vi "ReversedEngineering GetClassDependencyInfo.vi"(1 "Class/Create Path":path=path "C:/classes/P1S/EG1_class/EG1.lvclass", 5 "error in (no error)":errorcluster, 6 "AttributeSerachP{atternNamesToIgnore":string[](array[string]), 7 "Only analyse this class methods and attributes(False)":bool) -> (15 "classInfo":T5, 16 "TypeDefs":T1[](array[typedef]), 19 "error out":errorcluster)   [LabVIEW 2020]
doc: "Gets current diagram values"
uses:
  <resource>/Framework/Providers/Open_GDS/UML/ReversedEngineering/ReversedEngineering ClassInfoType.ctl
  <resource>/Framework/Providers/Open_GDS/ClassProviders/Common/CommonVIs/CommonVIs_VisibilityType.ctl
  <resource>/Framework/Providers/Open_GDS/ClassProviders/Common/CommonVIs/CommonVIs_AttributeInfoType.ctl
  <resource>/Framework/Providers/Open_GDS/ClassProviders/Common/CommonVIs/CommonVIs_AttributeDataType.ctl
  <resource>/Framework/Providers/Open_GDS/UML/ReversedEngineering/ReversedEngineering_ClassDependencyDetailsType.ctl
  <resource>/Framework/Providers/Open_GDS/ClassProviders/Common/ScriptingFunctions/SubVIs/Scripting_ViDependencyType.ctl
  <resource>/Framework/Providers/Open_GDS/ClassProviders/Common/CommonVIs/CommonVIs_TypeDefType.ctl
  <resource>/Framework/Providers/Open_GDS/ClassProviders/Provider_BaseClassInterface/ClassReader_class/MethodDependencyType.ctl
  <resource>/Framework/Providers/Open_GDS/UML/UMLEditor/UMLEditor BusyDialogAction.ctl
  <resource>/Framework/Providers/Open_GDS/ClassProviders/Provider_BaseClassInterface/ClassReader_class/ClassReader.lvclass
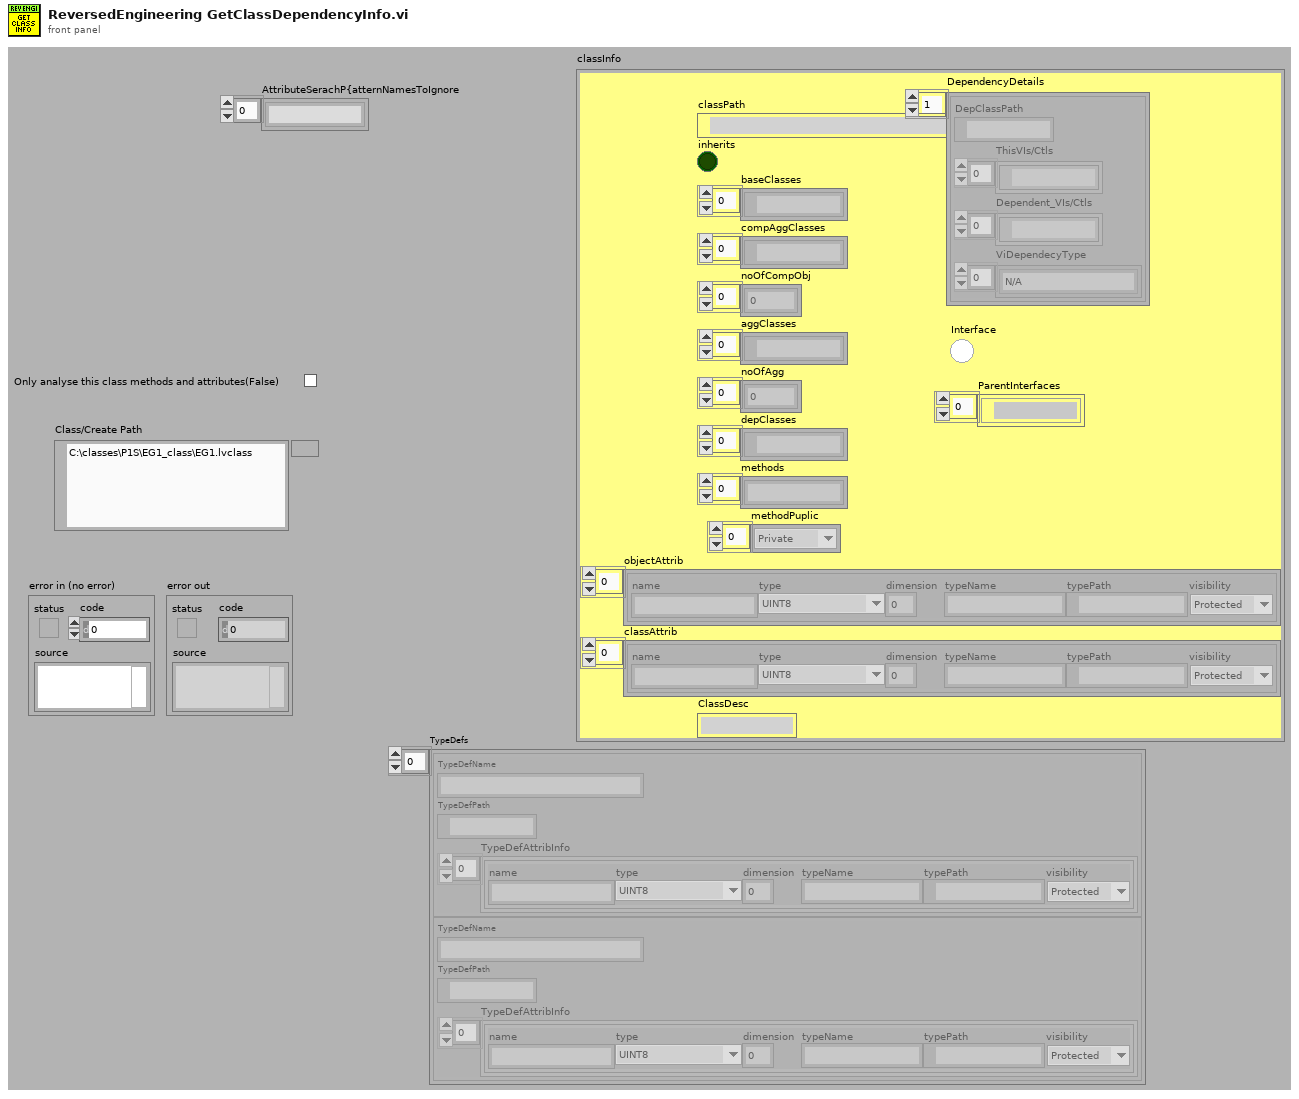
[diagram p1: front panel]
types:
  T1 = typedef "CommonVIs_TypeDefType.ctl" = cluster{"TypeDefName":string, "TypeDefPath":path, "TypeDefAttribInfo":T2[]}
  T2 = typedef "CommonVIs_AttributeInfoType.ctl" = cluster{"name":string, "type":T3, "dimension":i32, "typeName":string, "typePath":path, "visibility":T4}
  T3 = typedef "CommonVIs_AttributeDataType.ctl" = enum16{"UINT8", "INT8", "UINT16", "INT16", "UINT32", "INT32", "UINT64", "INT64", "SGL", "DBL", "EXT", "CSG", "CDB", "CXT", "TimeStamp", "STRING", "PATH", "BOOL", "ENUM", "RefNum", "VIRefNum", "LabVIEW Class", "Cluster", "Variant", "TypeDef", "Waveform", "LabVIEW Object", "Other", "void", "Set", "Map"}
  T4 = typedef "CommonVIs_VisibilityType.ctl" = enum16{"Public", "Private", "Protected"}
  T5 = typedef "ReversedEngineering ClassInfoType.ctl" = cluster{"classPath":path, "inherits":bool, "baseClasses":path[], "compAggClasses":path[], "noOfCompObj":i32[], "aggClasses":path[], "noOfAgg":i32[], "depClasses":path[], "methods":string[], "methodPuplic":T4[], "objectAttrib":T2[], "classAttrib":T2[], "ClassDesc":string, "DependencyDetails":T6[], "Interface":bool, "ParentInterfaces":path[]}
  T6 = typedef "ReversedEngineering_ClassDependencyDetailsType.ctl" = cluster{"DepClassPath":path, "ThisVIs/Ctls":path[], "Dependent_VIs/Ctls":path[], "ViDependecyType":T7[]}
  T7 = typedef "Scripting_ViDependencyType.ctl" = enum16{"N/A", "Launches"}
  T8 = typedef "ClassReader.lvclass/MethodDependencyType.ctl" = cluster{"Method/VI":path, "SubVIs/Ctls":path[], "SubVIClassOwner":string[], "ClassMethodName":string[], "SubVIClassOwnerPath":path[], "DepType":T7[]}
  T9 = cluster{"inherits":bool, "baseClasses":path[], "compositeAggregationClassPath":path[], "noOfCompositeObjects":i32[], "aggregationClassPath":path[], "noOfAggObjects":i32[], "dependencyClassPath":path[], "className":string, "classPath":path, "createRef":refnum<vi>, "depClassDescRefs":refnum<vi>[], "createPath":path, "depClassNames":string[], "depClassPaths":path[], "noOfObjects1":i32[], "refData":string, "refType":i16[], "noOfObjects2":i32[], "depTypeDefsVIs":path[], "depTypeDefsClassPath":path[], "depCreateClassPaths":path[], "objectRefsInAttrib":path[], "objectRefClassesInAttrib":path[], "objectRefInAttribIsAnArray":bool[], "methodNames":string[], "objectAttribInfo":T2[], "classAttribInfo":T2[], "errMsg":string, "dirClass":bool, "CreateClassVIsCalled":path[], "TypeDefs":T1[], "ClassDesc":string, "DependencyDetails":T6[], "methodPuplic":T4[], "depMethodVIs":T8[], "DataFlowClass":bool, "IsDependencyClassPathsAByValueClass":bool[], "Interface":bool, "ParentInterfaces":path[]}
  T10 = typedef "UMLEditor BusyDialogAction.ctl" = enum16{"Initialize", "Open(VIs)", "Open(i)", "Send_I-Value", "SendStatusMessage", "GetBusyDialogStatus", "Close", "Quit"}
  T11 = enum16{"NormalSubVis", "LV-Internal VIs", "All VIs", "All Functions"}
  T12 = enum32{"invalid VI type", "Standard VI", "Control VI", "Global VI", "Polymorphic VI", "Configuration VI", "SubSystem", "Facade VI", "Method VI", "Statechart Diagram VI"}
  T13 = enum32{"invalid scope", "public", "private", "protected", "community"}
  T14 = typedef "ClassTypes_MethodType.ctl" = cluster{"MethodName":string, "Visibility":enum16{"Public", "Private", "Protected"}, "StereoType":string, "Path":path}
  T15 = typedef "Librarian File Info Out.ctl" = cluster{"creation date":u32, "last mod date":u32, "type":string, "creator":string, "LV version":i32, "size":i32, "top level":bool}
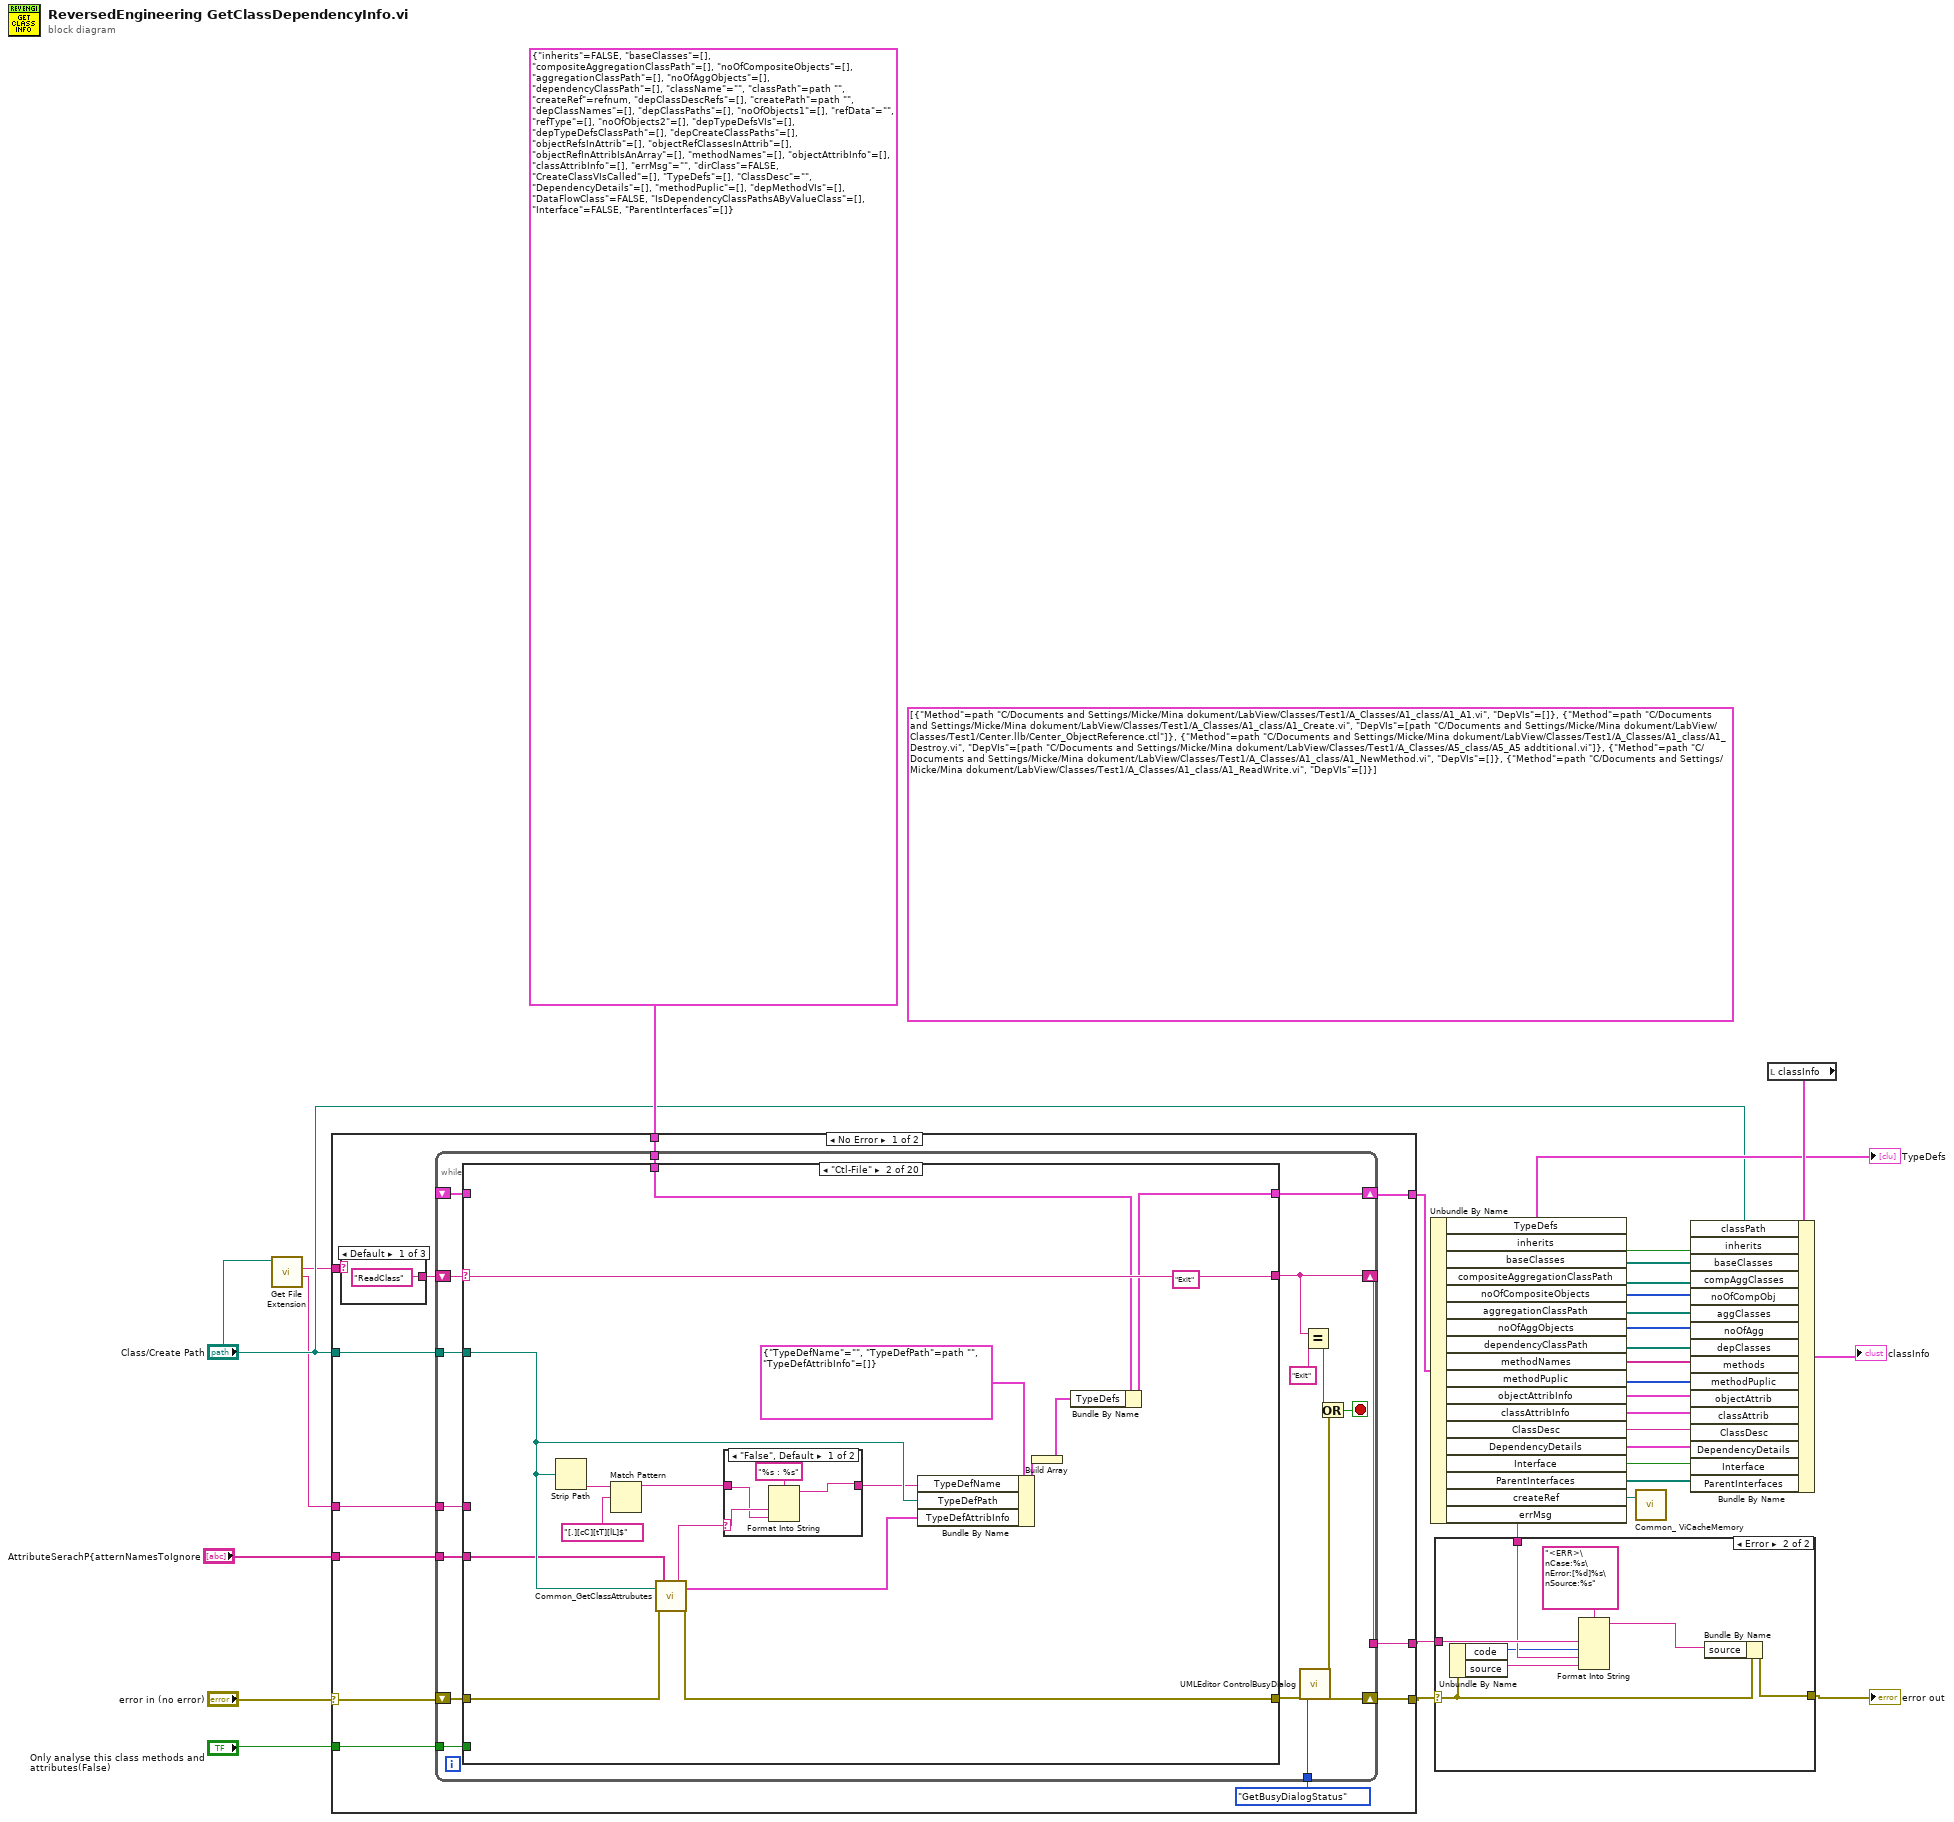
[diagram p0: block diagram]
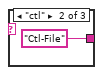
[diagram p3: hidden frame]
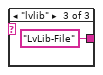
[diagram p4: hidden frame]
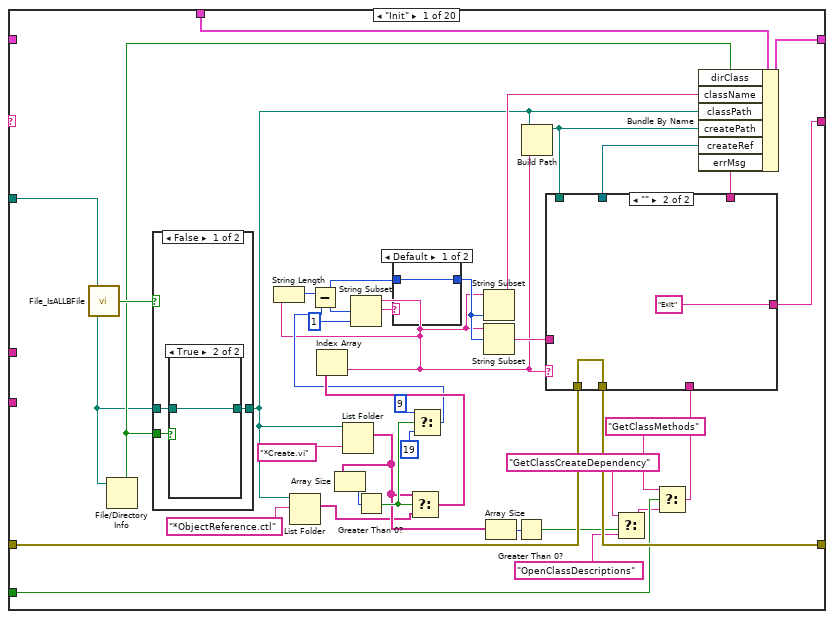
[diagram p5: hidden frame]
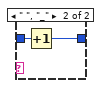
[diagram p6: hidden frame]
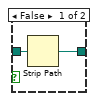
[diagram p7: hidden frame]
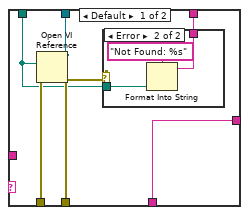
[diagram p9: hidden frame]
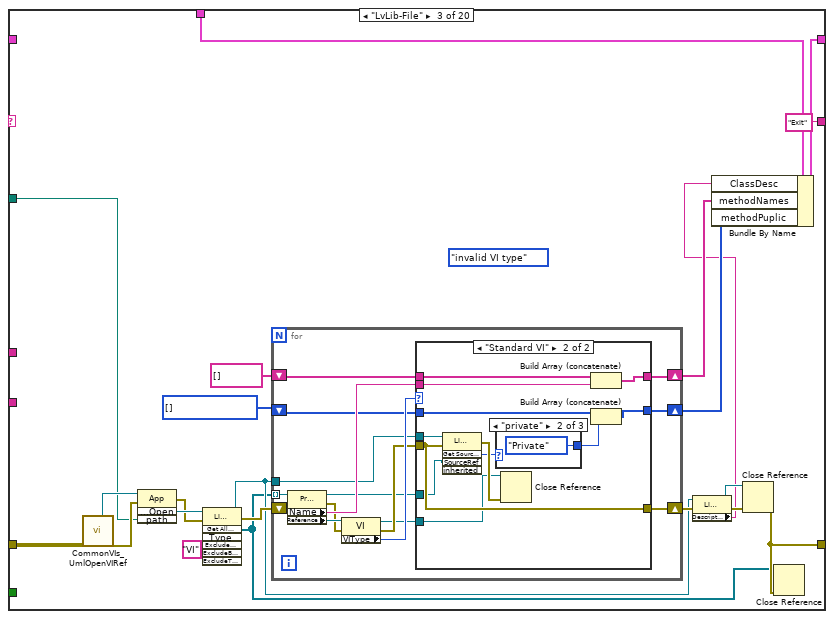
[diagram p12: hidden frame]
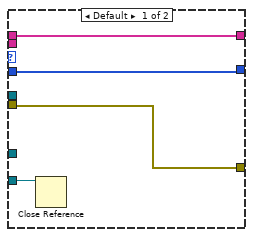
[diagram p13: hidden frame]
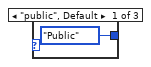
[diagram p14: hidden frame]
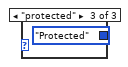
[diagram p15: hidden frame]
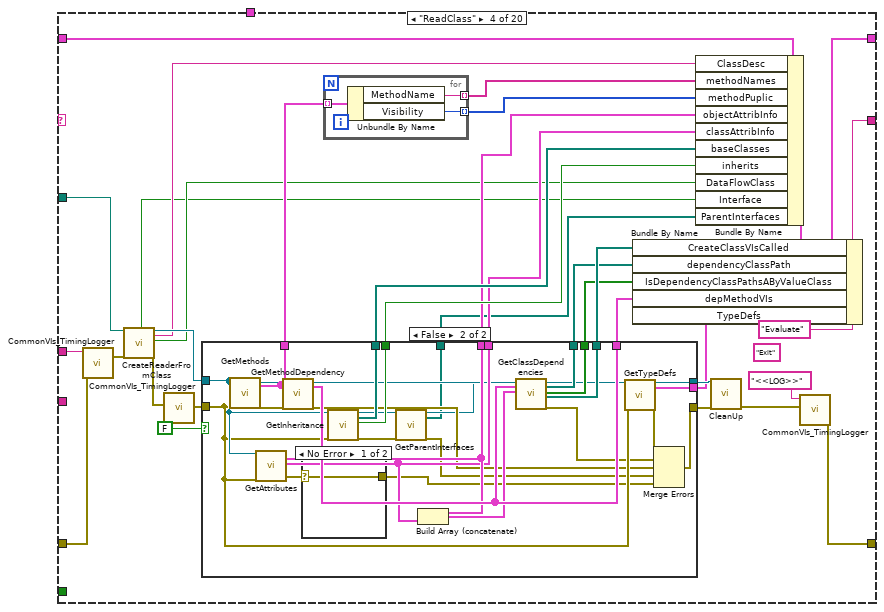
[diagram p16: hidden frame]
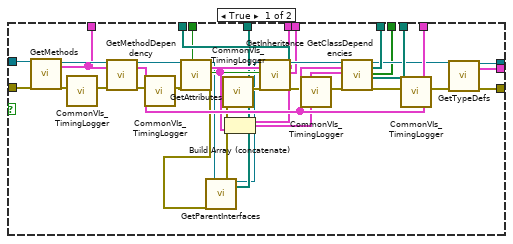
[diagram p17: hidden frame]
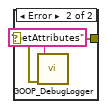
[diagram p18: hidden frame]
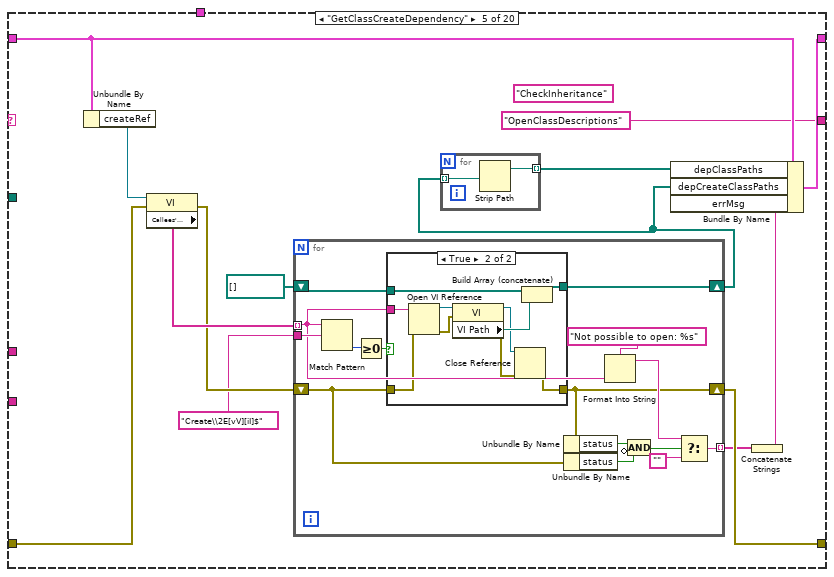
[diagram p19: hidden frame]
diagram:
  (unwired) cluster{"Method":path, "DepVIs":path[]}[] [{"Method"=path "C:/Documents and Settings/Micke/Mina dokument/LabView/Classes/Test1/A_Classes/A1_class/A1_A1.vi", "DepVIs"=[]}, {"Method"=path "C:/Documents and Settings/Micke/Mina dokument/LabView/Classes/Test1/A_Classes/A1_class/A1_Create.vi", "DepVIs"=[path "C:/Documents and Settings/Micke/Mina dokument/LabView/Classes/Test1/Center.llb/Center_ObjectReference.ctl"]}, {"Method"=path "C:/Documents and Settings/Micke/Mina dokument/LabView/Classes/Test1/A_Classes/A1_class/A1_Destroy.vi", "DepVIs"=[path "C:/Documents and Settings/Micke/Mina dokument/LabView/Classes/Test1/A_Classes/A5_class/A5_A5 addtitional.vi"]}, {"Method"=path "C:/Documents and Settings/Micke/Mina dokument/LabView/Classes/Test1/A_Classes/A1_class/A1_NewMethod.vi", "DepVIs"=[]}, {"Method"=path "C:/Documents and Settings/Micke/Mina dokument/LabView/Classes/Test1/A_Classes/A1_class/A1_ReadWrite.vi", "DepVIs"=[]}] ("depMethodVIs")
  n1 = call <vilib>:"Get File Extension.vi"("file"="Class/Create Path") -> ("filename without extension"=w4:string, "lowercase file extension"=w5:string)  [unwired: 1 in, 8 out]
  n2 = case shown="No Error" "error in (no error)" {
    selector: "error in (no error)" -> [w43 w1104]
    tunnel: [w42 w1104] -> w16
    tunnel: "Class/Create Path" -> [w41 _]
    tunnel: [w40 _] -> w30
    tunnel: [w39 _] -> w14
    tunnel: "Only analyse this class methods and attributes(False)" -> [w38 _]
    tunnel: T9 {"inherits"=FALSE, "baseClasses"=[], "compositeAggregationClassPath"=[], "noOfCompositeObjects"=[], "aggregationClassPath"=[], "noOfAggObjects"=[], "dependencyClassPath"=[], "className"="", "classPath"=path "", "createRef"=refnum, "depClassDescRefs"=[], "createPath"=path "", "depClassNames"=[], "depClassPaths"=[], "noOfObjects1"=[], "refData"="", "refType"=[], "noOfObjects2"=[], "depTypeDefsVIs"=[], "depTypeDefsClassPath"=[], "depCreateClassPaths"=[], "objectRefsInAttrib"=[], "objectRefClassesInAttrib"=[], "objectRefInAttribIsAnArray"=[], "methodNames"=[], "objectAttribInfo"=[], "classAttribInfo"=[], "errMsg"="", "dirClass"=FALSE, "CreateClassVIsCalled"=[], "TypeDefs"=[], "ClassDesc"="", "DependencyDetails"=[], "methodPuplic"=[], "depMethodVIs"=[], "DataFlowClass"=FALSE, "IsDependencyClassPathsAByValueClass"=[], "Interface"=FALSE, "ParentInterfaces"=[]} ("Cluster") -> [w36 _]
    tunnel: w5 -> [w35 _]
    tunnel: w4 -> [w33 _]
    tunnel: "AttributeSerachP{atternNamesToIgnore" -> [w32 _]
    frame No Error {
      n3 = case shown="Default" w35 {
        tunnel: ["ReadClass" ("y") "Ctl-File" "LvLib-File"] -> w34
        frame Default {
        }
        frame "ctl" {
        }
        frame "lvlib" {
        }
      }
      n4 = while {
        shift-right: [w61] -> _
        shift-left: w34 -> [w54]
        shift-right: [w48] -> w42
        shift-left: w43 -> [w62]
        shift-right: [w56] -> w40
        shift-left: _ -> [w57]
        tunnel: w41 -> [w55]
        tunnel: [w54] -> w39
        tunnel: w38 -> [w53]
        tunnel: UMLEditor_BusyDialogAction."GetBusyDialogStatus" ("Action(SendStatusMessage)") -> [w51]
        tunnel: w36 -> [w50]
        tunnel: w33 -> [w49]
        tunnel: w32 -> [w47]
        stop <- w58 stop-if-true
        n5 = case shown="\"Ctl-File\"" w54 {
          tunnel: w62 -> [w90 w137 w160 w206 w310 w344 w372 w437 w483 w579 w665 w685 w707 w730 w795 w817 w883 w958 w1022 w1101]
          tunnel: [w89 w135 w144 w200 w306 w340 w373 w437 w464 w579 w670 w698 w705 w730 w795 w817 w883 w958 w1022 w1101] -> w52
          tunnel: [w99 "Exit" ("y") "Exit" ("y") "Evaluate" ("y") "OpenClassDescriptions" ("y") "CheckInheritance" ("y") "GetMultiplicity" ("y") "GetClassMethods" ("y") "GetClassMethodDepenencies" ("y") "GetObjectAttributsDepenencies" ("y") "GetClassAttributsDepenencies" ("y") "CloseRefs" ("y") "Evaluate" ("y") "RemoveInheritDependency" ("y") "CreateTypeDefs?" ("y") "AddReferencedTypeDefs" ("y") "UpdateTypeDefsAttribName?" ("y") "SortMethodToClassDependencies" ("y") "Exit" ("y") "Exit" ("y")] -> w61
          tunnel: w57 -> [_ _ _ w229 w305 w362 w369 w440 w478 w575 w672 w693 w706 w714 w793 w812 w885 w965 w1021 w1103]
          tunnel: [w98 w134 w162 w220 w304 w363 w377 w442 w479 w580 w673 w694 w706 w729 w794 w819 w884 w964 w1023 w1103] -> w56
          tunnel: w55 -> [w71 w130 w159 w230 _ _ _ _ _ _ _ _ _ _ _ _ _ _ _ _]
          tunnel: w53 -> [w74 _ _ _ _ _ _ _ _ _ _ _ _ _ _ _ _ _ _ _]
          tunnel: w50 -> [w63 w126 w145 _ _ _ _ _ _ _ _ _ _ _ _ _ _ _ _ _]
          tunnel: w49 -> [_ _ _ w205 _ _ _ _ _ _ _ _ _ _ _ _ _ _ _ _]
          tunnel: w47 -> [_ w122 _ _ _ _ _ _ _ _ _ _ _ _ _ _ _ _ _ _]
          frame "Init" {
            n6 = call <resource>:"File_IsALLBFile.vi"("path"=w71) -> ("path to VI library?"=w100:bool)
            n7 = File/Directory Info(path=w71) -> (directory=w87:bool)  [unwired: 1 in, 6 out]
            n8 = case shown="False" w100 {
              tunnel: w71 -> [w106 w110]
              tunnel: [w105 w110] -> w67
              tunnel: w87 -> [w104 _]
              frame False {
                n9 = case shown="True" w104 {
                  tunnel: w106 -> [w108 w109]
                  tunnel: [w107 w109] -> w105
                  frame False {
                    n10 = Strip Path(path=w108) -> (stripped path=w107:path)  [unwired: 1 out]
                  }
                  frame True {
                  }
                }
              }
              frame True {
              }
            }
            n11 = List Folder(path=w67, pattern="*ObjectReference.ctl") -> (filenames=w65:string[])  [unwired: 1 in, 4 out]
            n12 = List Folder(path=w67, pattern="*Create.vi") -> (filenames=w70:string[])  [unwired: 1 in, 4 out]
            n13 = Array Size(array=w70) -> (size(s)=w84:i32)
            n14 = Greater Than 0?(x=w84) -> (x > 0?=w82:bool)
            n15 = Select(t=w70, s=w82, f=w65) -> (s? t:f=w83:string[])
            n16 = Index Array(array=w83) -> (element=w68:string)  [unwired: 1 in]
            n17 = String Length(string=w68) -> (length=w86:i32)
            n18 = Select(t=9 ("y"), s=w82, f=19 ("y")) -> (s? t:f=w79:i32)
            n19 = Subtract(x=w86, y=w79) -> (x-y=w85:i32)
            n20 = String Subset(string=w68, offset (0)=w85, length (rest)=1 ("length (rest)")) -> (substring=w92:string)
            n21 = case shown="Default" w92 {
              tunnel: w85 -> [w101 w103]
              tunnel: [w101 w102] -> w91
              frame Default {
              }
              frame " ", "_" {
                n22 = Increment(x=w103) -> (x+1=w102:i32)
              }
            }
            n23 = String Subset(string=w68, length (rest)=w91) -> (substring=w97:string)  [unwired: 1 out]
            n24 = String Subset(string=w68, offset (0)=w91) -> (substring=w94:string)  [unwired: 1 out]
            n25 = Array Size(array=w70) -> (size(s)=w78:i32)
            n26 = Greater Than 0?(x=w78) -> (x > 0?=w77:bool)
            n27 = Build Path(base path=w67, name or relative path=w68) -> (appended path=w96:path)
            n28 = Select(t="GetClassCreateDependency", s=w77, f="OpenClassDescriptions" ("y")) -> (s? t:f=w73:string)
            n29 = Select(t="GetClassMethods" ("y"), s=w74, f=w73) -> (s? t:f=w72:string)
            n30 = case shown="\"\"" w68 {
              tunnel: [w111 "Exit"] -> w99
              tunnel: w96 -> [w113 _]
              tunnel: [w116 _] -> w95
              tunnel: w94 -> [_ _]
              tunnel: w90 -> [w115 w120]
              tunnel: [w114 w120] -> w89
              tunnel: [w112 _] -> w88
              tunnel: w72 -> [w111 _]
              frame Default {
                n31 = Open VI Reference(vi path=w113, error in (no error)=w115) -> (vi reference=w116:refnum<vi>, error out=w114:errorcluster)  [unwired: 4 out]
                n32 = case shown="Error" w114 {
                  tunnel: w113 -> [_ w118]
                  tunnel: [_ w117] -> w112
                  frame No Error {
                  }
                  frame Error {
                    n33 = Format Into String(format string="Not Found: %s", w118) -> (resulting string=w117:string)  [unwired: 2 in, 1 out]
                  }
                }
              }
              frame "" {
              }
            }
            n34 = Bundle By Name(cluster=w63, "dirClass"=w87, "className"=w97, "classPath"=w67, "createPath"=w96, "createRef"=w95, "errMsg"=w88) -> (w98:T9)
          }
          frame "Ctl-File" {
            n35 = Strip Path(path=w130) -> (name=w132:string)  [unwired: 1 out]
            n36 = Match Pattern(string=w132, regular expression="[.][cC][tT][lL]$") -> (before substring=w124:string)  [unwired: 4 out]
            n37 = call <resource>:"Common_GetClassAttrubutes.vi"("Path(CtrlRenumf used if Path is empty)"=w130, "error in (no error)"=w137, "AttributeSerachP{atternNamesToIgnore"=w122) -> ("LibraryName"=w125:string, "attributeInfo"=w129:T2[], "error out"=w135:errorcluster)  [unwired: 1 in, 13 out]
            n38 = case shown="\"False\", Default" w125 {
              selector: w125 -> [w140 _]
              tunnel: w124 -> [w138 w142]
              tunnel: [w139 w142] -> w123
              frame "False", Default {
                n39 = Format Into String(format string="%s : %s", w140, w138) -> (resulting string=w139:string)  [unwired: 2 in, 1 out]
              }
              frame "" {
              }
            }
            n40 = Bundle By Name(cluster=T1 {"TypeDefName"="", "TypeDefPath"=path "", "TypeDefAttribInfo"=[]} ("TypeDef"), "TypeDefName"=w123, "TypeDefPath"=w130, "TypeDefAttribInfo"=w129) -> (w128:T1)
            n41 = Build Array(w128) -> (w127:T1[])
            n42 = Bundle By Name(cluster=w126, "TypeDefs"=w127) -> (w134:T9)
          }
          frame "LvLib-File" {
            (unwired) T12."invalid VI type" ("VI Type")
            w153 = T4[] [] items=["Public", "Private", "Protected"]
            n43 = call <resource>:"CommonVIs_UmlOpenVIRef.vi"("error in"=w160) -> ("AppRefOut"=w161:refnum<vi>)  [unwired: 3 in, 7 out]
            n44 = invoke class="App" method="Library.Open"(reference=w161, error in=w160, "path"=w159) -> (error out=w156:errorcluster, "Open Library"=w158:refnum<vi>)  [unwired: 1 in, 2 out]
            n45 = invoke class="Library" method="Get All Descendents"(reference=w158, error in=w156, "Type"="VI") -> (reference out=w147:refnum<vi>, error out=w155:errorcluster, "All Descendents"=w143:refnum<vi>[])  [unwired: 4 in, 4 out]
            n46 = for {
              tunnel: w143 -> [w178] mode=indexing
              shift-right: [w168] -> w150
              shift-left: w155 -> [w177]
              shift-right: [w173] -> w152
              shift-left: string[] [] -> [w174]
              tunnel: w147 -> [w166]
              shift-right: [w170] -> w151
              shift-left: w153 -> [w171]
              n47 = property class="ProjectItem"(reference=w178, error in=w177) -> (reference out=w164:refnum<vi>, error out=w165:errorcluster, "Name"=w172:string, "Reference"=w176:refnum<vi>)
              n48 = property class="VI"(reference=w176, error in=w165) -> (reference out=w167:refnum<vi>, error out=w169:errorcluster, "VIType"=w175:T12)
              n49 = case shown="\"Standard VI\"" w175 {
                tunnel: w174 -> [w182 w194]
                tunnel: [w182 w191] -> w173
                tunnel: w172 -> [_ w193]
                tunnel: w171 -> [w181 w192]
                tunnel: [w181 w190] -> w170
                tunnel: w169 -> [w180 w187]
                tunnel: [w180 w187] -> w168
                tunnel: w167 -> [w179 w184]
                tunnel: w166 -> [_ w186]
                tunnel: w164 -> [_ w183]
                frame Default {
                  n50 = Close Reference(reference=w179) -> ()  [unwired: 1 in, 1 out]
                }
                frame "Standard VI" {
                  n51 = invoke class="Library" method="Get Source Scope"(reference=w186, error in=w187, "SourceRef"=w183) -> (error out=w189:errorcluster, "GetSourceScope"=w188:T13)  [unwired: 2 in, 3 out]
                  n52 = case shown="\"private\"" w188 {
                    tunnel: [CommonVIs_VisibilityType."Public" ("Enum") CommonVIs_VisibilityType."Private" ("Enum") CommonVIs_VisibilityType."Protected" ("Enum")] -> w185
                    frame "public", Default {
                    }
                    frame "private" {
                    }
                    frame "protected" {
                    }
                  }
                  n53 = Close Reference(reference=w184, error in (no error)=w189) -> ()  [unwired: 1 out]
                  n54 = Build Array (concatenate)(w194, w193) -> (w191:string[])
                  n55 = Build Array (concatenate)(w192, w185) -> (w190:T4[])
                }
              }
            }
            n56 = property class="Library"(reference=w147, error in=w150) -> (reference out=w148:refnum<vi>, error out=w149:errorcluster, "Description"=w146:string)
            n57 = Bundle By Name(cluster=w145, "ClassDesc"=w146, "methodNames"=w152, "methodPuplic"=w151) -> (w162:T9)
            n58 = Close Reference(reference=w148, error in (no error)=w149) -> (error out=w144:errorcluster)
            n59 = Close Reference(reference=w143, error in (no error)=w144) -> ()  [unwired: 1 out]
          }
          frame "ReadClass" {
            (unwired) "Exit" ("y")
            n60 = call <resource>:"CommonVIs_TimingLogger.vi"("error in (no error)"=w206, "Name"=w205) -> ("error out"=w207:errorcluster)  [unwired: 9 in]
            n61 = call <resource>:"CreateReaderFromClass.vi"("ClassPath/LvClassRef"=w230, "error in"=w207) -> ("Is Interface"=w199:bool, "ClassReader"=w228:refnum<class "ClassReader.lvclass">, "Description"=w227:string, "DataFlowClass"=w213:bool, "error out"=w204:errorcluster)  [unwired: 13 out]
            n62 = call <resource>:"CommonVIs_TimingLogger.vi"("error in (no error)"=w204) -> ("error out"=w203:errorcluster)  [unwired: 10 in]
            n63 = case shown="False" FALSE {
              tunnel: w203 -> [w263 w277]
              tunnel: w228 -> [w262 w279]
              tunnel: [w261 w290] -> w224
              tunnel: [w260 w289] -> w223
              tunnel: [w258 w288] -> w222
              tunnel: [w255 w287] -> w219
              tunnel: [w254 w286] -> w218
              tunnel: [w253 w285] -> w217
              tunnel: [w252 w284] -> w215
              tunnel: [w251 w283] -> w214
              tunnel: [w248 w282] -> w212
              tunnel: [w247 w278] -> w211
              tunnel: [w246 w281] -> w210
              tunnel: [w245 w280] -> w209
              tunnel: [w233 w264] -> w198
              frame True {
                n64 = call-dynamic "GetMethods.vi"("ClassReader in"=w262, "error in (no error)"=w263) -> ("ClassReader out"=w259:refnum<class "ClassReader.lvclass">, "Methods"=w258:T14[], "error out"=w244:errorcluster)  [unwired: 15 out]
                n65 = call <resource>:"CommonVIs_TimingLogger.vi"("error in (no error)"=w244) -> ("error out"=w243:errorcluster)  [unwired: 10 in]
                n66 = call-dynamic "GetMethodDependency.vi"("ClassReader in"=w259, "Method(s)"=w258, "error in (no error)"=w243) -> ("ClassReader out"=w257:refnum<class "ClassReader.lvclass">, "DependencyVIs"=w253:T8[], "error out"=w242:errorcluster)  [unwired: 14 out]
                n67 = call <resource>:"CommonVIs_TimingLogger.vi"("error in (no error)"=w242) -> ("error out"=w241:errorcluster)  [unwired: 10 in]
                n68 = call-dynamic "GetAttributes.vi"("ClassReader in"=w257, "error in (no error)"=w241) -> ("ClassReader out"=w232:refnum<class "ClassReader.lvclass">, "ObjectAttributes"=w252:T2[], "ClassAttributes"=w251:T2[], "error out"=w235:errorcluster)  [unwired: 1 in, 13 out]
                n69 = call-dynamic "GetParentInterfaces.vi"("ClassReader in"=w232, "error in (no error)"=w235) -> ("ClassReader out"=w231:refnum<class "ClassReader.lvclass">, "ParentInterfaces"=w233:path[], "error out"=w234:errorcluster)  [unwired: 15 in]
                n70 = call <resource>:"CommonVIs_TimingLogger.vi"("error in (no error)"=w234) -> ("error out"=w240:errorcluster)  [unwired: 10 in]
                n71 = Build Array (concatenate)(w252, w251) -> (w250:T2[])
                n72 = call-dynamic "GetInheritance.vi"("ClassReader in"=w231, "error in (no error)"=w240) -> ("ClassReader out"=w256:refnum<class "ClassReader.lvclass">, "Inheritance"=w261:path[], "Inherits"=w260:bool, "error out"=w238:errorcluster)  [unwired: 14 out]
                n73 = call <resource>:"CommonVIs_TimingLogger.vi"("error in (no error)"=w238) -> ("error out"=w239:errorcluster)  [unwired: 10 in]
                n74 = call-dynamic "GetClassDependencies.vi"("ClassReader in"=w256, "DependencyVIs"=w253, "Attributes"=w250, "error in (no error)"=w239) -> ("ClassReader out"=w249:refnum<class "ClassReader.lvclass">, "DependencyClassPaths"=w254:path[], "IsDependencyClassPathsAByValueClass"=w245:bool[], "CreateClassVIsCalled"=w255:path[], "error out"=w237:errorcluster)  [unwired: 11 out]
                n75 = call <resource>:"CommonVIs_TimingLogger.vi"("error in (no error)"=w237) -> ("error out"=w236:errorcluster)  [unwired: 10 in]
                n76 = call-dynamic "GetTypeDefs.vi"("ClassReader in"=w249, "error in (no error)"=w236) -> ("ClassReader out"=w248:refnum<class "ClassReader.lvclass">, "TypeDefs"=w246:T1[], "error out"=w247:errorcluster)  [unwired: 15 out]
              }
              frame False {
                n77 = call-dynamic "GetMethods.vi"("ClassReader in"=w279, "error in (no error)"=w277) -> ("ClassReader out"=w276:refnum<class "ClassReader.lvclass">, "Methods"=w288:T14[], "error out"=w275:errorcluster)  [unwired: 15 out]
                n78 = call-dynamic "GetAttributes.vi"("ClassReader in"=w279, "error in (no error)"=w277) -> ("ObjectAttributes"=w284:T2[], "ClassAttributes"=w283:T2[], "error out"=w272:errorcluster)  [unwired: 1 in, 14 out]
                n79 = call-dynamic "GetMethodDependency.vi"("ClassReader in"=w276, "Method(s)"=w288, "error in (no error)"=w275) -> ("DependencyVIs"=w285:T8[], "error out"=w270:errorcluster)  [unwired: 15 out]
                n80 = case shown="No Error" w272 {
                  selector: w272 -> [w291 w293]
                  tunnel: [w291 w293] -> w269
                  frame No Error {
                  }
                  frame Error {
                    n81 = call <resource>:"GOOP_DebugLogger.vi"("error in (no error)"=w293, "State"="GetAttributes") -> ()  [unwired: 7 in, 3 out]
                  }
                }
                n82 = call-dynamic "GetInheritance.vi"("ClassReader in"=w279, "error in (no error)"=w277) -> ("ClassReader out"=w267:refnum<class "ClassReader.lvclass">, "Inheritance"=w290:path[], "Inherits"=w289:bool, "error out"=w268:errorcluster)  [unwired: 14 out]
                n83 = call-dynamic "GetParentInterfaces.vi"("ClassReader in"=w267, "error in (no error)"=w268) -> ("ClassReader out"=w266:refnum<class "ClassReader.lvclass">, "ParentInterfaces"=w264:path[], "error out"=w265:errorcluster)  [unwired: 15 in]
                n84 = Build Array (concatenate)(w284, w283) -> (w273:T2[])
                n85 = call-dynamic "GetClassDependencies.vi"("ClassReader in"=w266, "DependencyVIs"=w285, "Attributes"=w273) -> ("DependencyClassPaths"=w286:path[], "IsDependencyClassPathsAByValueClass"=w280:bool[], "CreateClassVIsCalled"=w287:path[], "error out"=w271:errorcluster)  [unwired: 1 in, 12 out]
                n86 = call-dynamic "GetTypeDefs.vi"("ClassReader in"=w279, "error in (no error)"=w277) -> ("ClassReader out"=w282:refnum<class "ClassReader.lvclass">, "TypeDefs"=w281:T1[], "error out"=w274:errorcluster)  [unwired: 15 out]
                n87 = Merge Errors(w274, w271, w270, w265, w269) -> (w278:errorcluster)
              }
            }
            n88 = for {
              tunnel: w222 -> [w296] mode=indexing
              tunnel: [w295] -> w226 mode=indexing
              tunnel: [w294] -> w225 mode=indexing
              n89 = Unbundle By Name(w296) -> ("MethodName"=w295:string, "Visibility"=w294:enum16{"Public", "Private", "Protected"})
            }
            n90 = Bundle By Name(cluster=w229, "ClassDesc"=w227, "methodNames"=w226, "methodPuplic"=w225, "objectAttribInfo"=w215, "classAttribInfo"=w214, "baseClasses"=w224, "inherits"=w223, "DataFlowClass"=w213, "Interface"=w199, "ParentInterfaces"=w198) -> (w221:T9)
            n91 = Bundle By Name(cluster=w221, "CreateClassVIsCalled"=w219, "dependencyClassPath"=w218, "IsDependencyClassPathsAByValueClass"=w209, "depMethodVIs"=w217, "TypeDefs"=w210) -> (w220:T9)
            n92 = call-dynamic "CleanUp.vi"("reference in"=w212, "error in (no error)"=w211) -> ("error out"=w201:errorcluster)  [unwired: 17 out]
            n93 = call <resource>:"CommonVIs_TimingLogger.vi"("error in (no error)"=w201, "Name"="<<LOG>>") -> ("error out"=w200:errorcluster)  [unwired: 9 in]
          }
          frame "GetClassCreateDependency" {
            (unwired) "CheckInheritance" ("y")
            n94 = Unbundle By Name(w305) -> ("createRef"=w298:refnum<vi>)
            n95 = property class="VI"(reference=w298, error in=w310) -> (error out=w308:errorcluster, "Callees' Names"=w309:string[])  [unwired: 1 out]
            n96 = for {
              tunnel: w309 -> [w313] mode=indexing
              shift-right: [w324] -> w300
              shift-left: path[] [] -> [w325]
              shift-right: [w316] -> w306
              shift-left: w308 -> [w315]
              tunnel: "Create\\2E[vV][iI]$" ("regular expression") -> [w323]
              tunnel: [w314] -> w301 mode=indexing
              n97 = Match Pattern(string=w313, regular expression=w323) -> (offset past match=w327:i32)  [unwired: 4 out]
              n98 = Greater Or Equal To 0?(x=w327) -> (x >= 0?=w326:bool)
              n99 = case shown="True" w326 {
                tunnel: w325 -> [w329 w339]
                tunnel: w313 -> [_ w338]
                tunnel: w315 -> [w328 w337]
                tunnel: [w329 w333] -> w324
                tunnel: [w328 w330] -> w316
                frame False {
                }
                frame True {
                  n100 = Open VI Reference(vi path=w338, error in (no error)=w337) -> (vi reference=w336:refnum<vi>, error out=w335:errorcluster)  [unwired: 1 in, 3 out]
                  n101 = property class="VI"(reference=w336, error in=w335) -> (reference out=w331:refnum<vi>, error out=w332:errorcluster, "VI Path"=w334:path)
                  n102 = Close Reference(reference=w331, error in (no error)=w332) -> (error out=w330:errorcluster)
                  n103 = Build Array (concatenate)(w339, w334) -> (w333:path[])
                }
              }
              n104 = Unbundle By Name(w316) -> ("status"=w322:bool)
              n105 = Unbundle By Name(w315) -> ("status"=w321:bool)
              n106 = Format Into String(format string="Not possible to open: %s", w313) -> (resulting string=w317:string)  [unwired: 2 in, 1 out]
              n107 = Compound Arithmetic op=AND(w322, invert w321) -> (w320:bool)
              n108 = Select(t=w317, s=w320, f="") -> (s? t:f=w314:string)
            }
            n109 = for {
              tunnel: w300 -> [w312] mode=indexing
              tunnel: [w311] -> w303 mode=indexing
              n110 = Strip Path(path=w312) -> (stripped path=w311:path)  [unwired: 1 out]
            }
            n111 = Concatenate Strings(w301) -> (w299:string)
            n112 = Bundle By Name(cluster=w305, "depClassPaths"=w303, "depCreateClassPaths"=w300, "errMsg"=w299) -> (w304:T9)
          }
          frame "OpenClassDescriptions" {
            n113 = Unbundle By Name(w362) -> ("classPath"=w348:path)
            n114 = call <resource>:"CommonVIs_ListFilesRecursive.vi"("directory path"=w348, "FileSearchPattern"="*ClassDescription.vi", "error in (no error)"=w344) -> ("Files"=w346:path[], "error out"=w343:errorcluster)  [unwired: 3 in, 12 out]
            n115 = Index Array(array=w346) -> (element=w345:path)  [unwired: 1 in]
            n116 = Open VI Reference(vi path=w345, error in (no error)=w343) -> (vi reference=w354:refnum<vi>, error out=w355:errorcluster)  [unwired: 1 in, 3 out]
            n117 = Unbundle By Name(w355) -> ("status"=w361:bool)
            n118 = Unbundle By Name(w343) -> ("status"=w360:bool)
            n119 = invoke class="VI" method="Ctrl Val.Get"(reference=w354, error in=w355, "Control Name"="Class description") -> (reference out=w341:refnum<vi>, error out=w342:errorcluster, "Get Control Value Variant"=w351:variant)  [unwired: 1 in, 1 out]
            n120 = Format Into String(format string="Not Found: %s", w345) -> (resulting string=w356:string)  [unwired: 2 in, 1 out]
            n121 = Compound Arithmetic op=AND(w361, invert w360) -> (w359:bool)
            n122 = Select(t=w356, s=w359, f="") -> (s? t:f=w350:string)
            n123 = Variant To Data(type=w350, Variant=w351) -> (data=w349:string)  [unwired: 1 in, 1 out]
            n124 = call <resource>:"Common_ ViCacheMemory.vi"("ViRef"=w341, "error in (no error)"=w342) -> ("error out"=w340:errorcluster)  [unwired: 2 in, 15 out]
            n125 = Bundle By Name(cluster=w362, "errMsg"=w350, "ClassDesc"=w349) -> (w363:T9)
          }
          frame "CheckInheritance" {
            n126 = Unbundle By Name(w369) -> ("dirClass"=w368:bool)  [unwired: 1 out]
            n127 = Unbundle By Name(w369) -> ("classPath"=w367:path, "className"=w380:string)
            n128 = Concatenate Strings(w380, "GOOPKernel.vi" ("string")) -> (w378:string)
            n129 = case shown="True" w368 {
              tunnel: w367 -> [w381 w384]
              tunnel: [w381 w383] -> w366
              tunnel: "private" ("element") -> [_ w382]
              frame False {
              }
              frame True {
                n130 = Build Path(base path=w384, name or relative path=w382) -> (appended path=w383:path)
              }
            }
            n131 = Build Path(base path=w366, name or relative path=w378) -> (appended path=w371:path)
            n132 = while {
              tunnel: [w391] -> w376 mode=indexing
              shift-right: [w390] -> w373
              shift-left: w372 -> [w392]
              tunnel: [w389] -> w364 mode=indexing
              shift-right: [w387] -> _
              shift-left: w371 -> [w388]
              shift-right: [w385] -> w370
              shift-left: w369 -> [w386]
              stop <- w391 continue-if-true
              n133 = Open VI Reference(vi path=w388, error in (no error)=w392) -> (vi reference=w399:refnum<vi>, error out=w398:errorcluster)  [unwired: 4 out]
              n134 = property class="VI"(reference=w399, error in=w398) -> (reference out=w389:refnum<vi>, error out=w393:errorcluster, "Callees' Names"=w397:string[])
              n135 = Array Size(array=w397) -> (size(s)=w395:i32)
              n136 = while {
                tunnel: w397 -> [w423] mode=indexing
                tunnel: "GOOPKernel.[vV][iI]$" ("string") -> [w430]
                tunnel: w395 -> [w421]
                tunnel: [w425] -> w391
                tunnel: [w424] -> _
                tunnel: [w423] -> w394
                i -> [w429]
                stop <- w426 stop-if-true
                n137 = Increment(x=w429) -> (x+1=w422:i32)
                n138 = Match Pattern(string=w423, regular expression=w430) -> (before substring=w424:string, offset past match=w428:i32)  [unwired: 3 out]
                n139 = Greater Or Equal?(x=w422, y=w421) -> (x >= y?=w427:bool)
                n140 = Greater Or Equal To 0?(x=w428) -> (x >= 0?=w425:bool)
                n141 = Or(x=w425, y=w427) -> (x .or. y?=w426:bool)
              }
              n142 = case shown="True" w391 {
                tunnel: w394 -> [_ w417]
                tunnel: w393 -> [w402 w412]
                tunnel: [w402 w411] -> w390
                tunnel: w386 -> [w401 w409]
                tunnel: [w401 w410] -> w385
                tunnel: [path "" ("Path") w406] -> w387
                frame False {
                }
                frame True {
                  # "Iheritance"
                  n143 = Unbundle By Name(w409) -> ("baseClasses"=w408:path[])
                  n144 = Open VI Reference(vi path=w417, error in (no error)=w412) -> (vi reference=w416:refnum<vi>, error out=w415:errorcluster)  [unwired: 4 out]
                  n145 = property class="VI"(reference=w416, error in=w415) -> (reference out=w414:refnum<vi>, error out=w413:errorcluster, "VI Path"=w406:path)
                  n146 = Strip Path(path=w406) -> (stripped path=w404:path)  [unwired: 1 out]
                  n147 = call <resource>:"File_IsALLBFile.vi"("path"=w404) -> ("path to VI library?"=w405:bool)
                  n148 = case shown="False" w405 {
                    tunnel: [w418 w420] -> w403
                    tunnel: w404 -> [w419 w420]
                    frame False {
                      n149 = Strip Path(path=w419) -> (stripped path=w418:path)  [unwired: 1 out]
                    }
                    frame True {
                    }
                  }
                  n150 = Build Array (concatenate)(w408, w403) -> (w407:path[])
                  n151 = Bundle By Name(cluster=w409, "baseClasses"=w407) -> (w410:T9)
                  n152 = Close Reference(reference=w414, error in (no error)=w413) -> (error out=w411:errorcluster)
                }
              }
            }
            n153 = Or Array Elements(Boolean array=w376) -> (logical OR=w374:bool)
            n154 = Bundle By Name(cluster=w370, "inherits"=w374) -> (w377:T9)
            n155 = call <resource>:"Common_ ViCacheMemory.vi"("ViRef-Array"=w364) -> ()  [unwired: 3 in, 16 out]
          }
          frame "GetMultiplicity" {
            n156 = Unbundle By Name(w440) -> ("depCreateClassPaths"=w445:path[], "createRef"=w446:refnum<vi>)
            n157 = Unbundle By Name(w440) -> ("baseClasses"=w439:path[])
            n158 = property class="VI"(reference=w446) -> ("Block Diagram"=w436:refnum<vi>)  [unwired: 1 in, 2 out]
            n159 = Index Array(array=w439) -> (element=w438:path)  [unwired: 1 in]
            n160 = call <resource>:"ReversedEngineering GetDiagramSubVIs.vi"("Diagram"=w436, "SubVIsOptions(NormalSubVis)"=T11."NormalSubVis", "RecrsiveSearchInNormalSubVIs(False)"=FALSE, "error in (no error)"=errorcluster {"status"=FALSE, "code"=0, "source"=""}, "PathToDebugVI(OnlyUsedForRecursivVitFiles)"=path "") -> ("DiagramOut"=w435:refnum<vi>, "SubViNames"=w444:string[])  [unwired: 13 out]
            n161 = Close Reference(reference=w435) -> ()  [unwired: 1 in, 1 out]
            n162 = for {
              tunnel: w445 -> [w448] mode=indexing
              tunnel: w444 -> [w455]
              tunnel: [w451] -> w443 mode=indexing
              tunnel: w438 -> [w450]
              n163 = Strip Path(path=w448) -> (stripped path=w447:path, name=w454:string)
              n164 = Equal?(x=w450, y=w447) -> (x = y?=w449:bool)
              n165 = for {
                tunnel: w455 -> [w462] mode=indexing
                tunnel: w454 -> [w461]
                tunnel: [w459] -> w453 mode=indexing
                n166 = Equal?(x=w461, y=w462) -> (x = y?=w460:bool)
                n167 = Boolean To (0,1)(Boolean=w460) -> (0, 1=w459:i16)
              }
              n168 = Add Array Elements(numeric array=w453) -> (sum=w452:i16)
              n169 = case shown="True" w449 {
                tunnel: w452 -> [w456 w458]
                tunnel: [w456 w457] -> w451
                frame False {
                }
                frame True {
                  n170 = Decrement(x=w458) -> (x-1=w457:i16)
                }
              }
            }
            n171 = Bundle By Name(cluster=w440, "noOfObjects1"=w443) -> (w442:T9)
          }
          frame "GetClassMethods" {
            w463 = T8[] []  # depMethodVIs
            n172 = Unbundle By Name(w478) -> ("className"=w470:string, "classPath"=w467:path)
            n173 = Unbundle By Name(w478) -> ("dirClass"=w472:bool, "classPath"=w471:path)
            n174 = List Folder(path=w467, pattern="*.vi", error in=w483) -> (path out=w486:path, filenames=w485:string[], error out=w480:errorcluster)  [unwired: 2 out]
            n175 = for {
              tunnel: w486 -> [w568]
              tunnel: w485 -> [w566] mode=indexing
              tunnel: [w567] -> w484 mode=indexing
              n176 = Build Path(base path=w568, name or relative path=w566) -> (appended path=w567:path)
            }
            n177 = case shown="False" w472 {
              tunnel: w471 -> [_ w493]
              tunnel: [path[] [] w490] -> w469
              frame False {
              }
              frame True {
                n178 = List Folder(path=w493) -> (path out=w492:path, folder names=w491:string[])  [unwired: 1 in, 4 out]
                n179 = for {
                  tunnel: w492 -> [w497]
                  tunnel: w491 -> [w494] mode=indexing
                  shift-right: [w495] -> w490
                  shift-left: path[] [] -> [w496]
                  n180 = case shown="Default" w494 {
                    tunnel: w497 -> [_ w504]
                    tunnel: w494 -> [_ w503]
                    tunnel: w496 -> [w498 w501]
                    tunnel: [w498 w500] -> w495
                    frame "Example", "Examples", "Test" {
                    }
                    frame Default {
                      n181 = Build Path(base path=w504, name or relative path=w503) -> (appended path=w502:path)
                      n182 = List Folder(path=w502, pattern="*.vi") -> (path out=w506:path, filenames=w507:string[])  [unwired: 1 in, 3 out]
                      n183 = for {
                        tunnel: w506 -> [w510]
                        tunnel: w507 -> [w508] mode=indexing
                        tunnel: [w509] -> w499 mode=indexing
                        n184 = Build Path(base path=w510, name or relative path=w508) -> (appended path=w509:path)
                      }
                      n185 = Build Array (concatenate)(w501, w499) -> (w500:path[])
                    }
                  }
                }
              }
            }
            n186 = Build Array (concatenate)(w484, w469) -> (w468:path[])
            n187 = call <resource>:"CommonVIs_HideClassMethods.vi"("Item Paths"=w468, "error in (no error)"=w480) -> ("Item Paths filtered"=w482:path[], "error out"=w481:errorcluster)  [unwired: 16 out]
            n188 = for {
              tunnel: w482 -> [w517] mode=indexing
              shift-right: [w522] -> w465
              shift-left: w481 -> [w538]
              shift-right: [w520] -> w477
              shift-left: w463 -> [w519]
              tunnel: [w514] -> w475 mode=indexing
              tunnel: "[.][vV][iI][tT]*$" ("regular expression") -> [w534]
              tunnel: [w533] -> w473 mode=indexing
              tunnel: w470 -> [w528]
              tunnel: w467 -> [w524]
              tunnel: [w523] -> w466 mode=indexing
              n189 = Strip Path(path=w517) -> (stripped path=w531:path, name=w529:string)
              n190 = call <resource>:"File_IsALLBFile.vi"("path"=w531) -> ("path to VI library?"=w532:bool)
              n191 = case shown="False" w532 {
                tunnel: [w541 w545] -> w515
                tunnel: w517 -> [_ w544]
                tunnel: w531 -> [w543 _]
                tunnel: w524 -> [w542 _]
                frame False {
                  n192 = Equal?(x=w543, y=w542) -> (x = y?=w541:bool)
                }
                frame True {
                  n193 = call <vilib>:"Get VI Library File Info.vi"("path"=w544) -> ("file information"=w546:T15)  [unwired: 1 in, 9 out]
                  n194 = Unbundle By Name(w546) -> ("top level"=w545:bool)
                }
              }
              n195 = Open VI Reference(vi path=w517, error in (no error)=w538) -> (vi reference=w540:refnum<vi>, error out=w539:errorcluster)  [unwired: 4 out]
              n196 = Match Pattern(string=w529, regular expression=w528) -> (before substring=w527:string, after substring=w526:string, offset past match=w530:i32)  [unwired: 2 out]
              n197 = property class="VI"(reference=w540, error in=w539) -> (reference out=w523:refnum<vi>, error out=w536:errorcluster, "Callees' Names"=w537:string[])
              n198 = Concatenate Strings(w527, w526) -> (w525:string)
              n199 = Match Pattern(string=w525, regular expression=w534, offset (0)=w530) -> (before substring=w533:string)  [unwired: 3 out]
              n200 = Select(t=CommonVIs_VisibilityType."Public" ("Enum"), s=w515, f=CommonVIs_VisibilityType."Private" ("Enum")) -> (s? t:f=w514:T4)
              n201 = for {
                tunnel: w537 -> [w547] mode=indexing
                shift-right: [w552] -> w522
                shift-left: w536 -> [w553]
                tunnel: "[.][~.]+$" ("regular expression") -> [w551]
                shift-right: [w548] -> w518
                shift-left: path[] [] -> [w549]
                n202 = Match Pattern(string=w547, regular expression=w551) -> (offset past match=w550:i32)  [unwired: 4 out]
                n203 = case shown="0.." w550 {
                  tunnel: w553 -> [w555 w565]
                  tunnel: [w555 w560] -> w552
                  tunnel: w547 -> [_ w559]
                  tunnel: w549 -> [w554 w557]
                  tunnel: [w554 w558] -> w548
                  frame Default {
                  }
                  frame 0.. {
                    n204 = Open VI Reference(vi path=w559, error in (no error)=w565) -> (vi reference=w562:refnum<vi>, error out=w561:errorcluster)  [unwired: 4 out]
                    n205 = property class="VI"(reference=w562, error in=w561) -> (reference out=w564:refnum<vi>, error out=w563:errorcluster, "VI Path"=w556:path)
                    n206 = Build Array (concatenate)(w557, w556) -> (w558:path[])
                    n207 = Close Reference(reference=w564, error in (no error)=w563) -> (error out=w560:errorcluster)
                  }
                }
              }
              n208 = Bundle(cluster=T8 {"Method/VI"=path "", "SubVIs/Ctls"=[], "SubVIClassOwner"=[], "ClassMethodName"=[], "SubVIClassOwnerPath"=[], "DepType"=[]}, "Method/VI"=w517, "SubVIs/Ctls"=w518) -> (w516:T8)  [unwired: 4 out]
              n209 = Build Array (concatenate)(w519, w516) -> (w520:T8[])
            }
            n210 = Bundle By Name(cluster=w478, "methodNames"=w473, "methodPuplic"=w475, "depMethodVIs"=w477) -> (w479:T9)
            n211 = call <resource>:"Common_ ViCacheMemory.vi"("ViRef-Array"=w466, "error in (no error)"=w465) -> ("error out"=w464:errorcluster)  [unwired: 2 in, 15 out]
          }
          frame "GetClassMethodDepenencies" {
            w570 = path[] []
            n212 = Unbundle By Name(w575) -> ("dirClass"=w577:bool, "classPath"=w576:path, "depMethodVIs"=w573:T8[])
            n213 = Unbundle By Name(w575) -> ("baseClasses"=w574:path[])
            n214 = for {
              tunnel: w577 -> [w593]
              tunnel: w576 -> [w592]
              tunnel: w574 -> [w591]
              tunnel: w573 -> [w581] mode=indexing
              shift-right: [w589] -> w572
              shift-left: w570 -> [w590]
              shift-right: [w588] -> w571
              shift-left: w570 -> [w587]
              tunnel: w570 -> [w585]
              tunnel: [w582] -> w569 mode=indexing
              n215 = Unbundle(w581) -> ("Method/VI"=w583:path, "SubVIs/Ctls"=w586:path[])  [unwired: 4 out]
              n216 = for {
                shift-right: [w632] -> w589
                shift-left: w590 -> [w633]
                tunnel: w593 -> [w626]
                tunnel: w592 -> [w625]
                shift-right: [w615] -> w588
                shift-left: w587 -> [w616]
                tunnel: w591 -> [w610]
                tunnel: w586 -> [w598] mode=indexing
                shift-right: [w597] -> w584
                shift-left: w585 -> [w599]
                w623 = "*GOOPKernel.vi" ("pattern")
                # "Its a Class Method"
                n217 = Strip Path(path=w598) -> (stripped path=w604:path, name=w614:string)
                n218 = Match Pattern(string=w614, regular expression="[Cc][Rr][Ee][Aa][Tt][Ee].vi$" ("string")) -> (offset past match=w612:i32)  [unwired: 4 out]
                n219 = for {
                  tunnel: w614 -> [w656]
                  tunnel: string[] ["ObjectAttributes.ctl$", "ClassAttributes.ctl$"] -> [w655] mode=indexing
                  tunnel: [w653] -> w628 mode=indexing
                  n220 = Match Pattern(string=w656, regular expression=w655) -> (offset past match=w654:i32)  [unwired: 4 out]
                  n221 = Greater Or Equal To 0?(x=w654) -> (x >= 0?=w653:bool)
                }
                n222 = List Folder(path=w604, pattern=w623) -> (filenames=w631:string[])  [unwired: 1 in, 4 out]
                n223 = Greater Or Equal To 0?(x=w612) -> (x >= 0?=w611:bool)
                n224 = Build Path(base path=w604, name or relative path="private" ("element")) -> (appended path=w624:path)
                n225 = Search 1D Array(1D array=w610, element=w604) -> (index of element=w609:i32)  [unwired: 1 out]
                n226 = List Folder(path=w624, pattern=w623) -> (filenames=w622:string[])  [unwired: 1 in, 4 out]
                n227 = Or Array Elements(Boolean array=w628) -> (logical OR=w627:bool)
                n228 = Array Size(array=w631) -> (size(s)=w630:i32)
                n229 = case shown="False" w626 {
                  tunnel: [w645 w650] -> w600
                  tunnel: w604 -> [w644 w652]
                  tunnel: w625 -> [w643 w646]
                  frame False {
                    n230 = Not Equal?(x=w643, y=w644) -> (x != y?=w645:bool)
                  }
                  frame True {
                    n231 = Not Equal?(x=w646, y=w652) -> (x != y?=w649:bool)
                    n232 = Build Path(base path=w646, name or relative path="private" ("element")) -> (appended path=w651:path)
                    n233 = Not Equal?(x=w651, y=w652) -> (x != y?=w648:bool)
                    n234 = And(x=w649, y=w648) -> (x .and. y?=w650:bool)
                  }
                }
                n235 = Search 1D Array(1D array=w633, element=w604) -> (index of element=w634:i32)  [unwired: 1 out]
                n236 = Array Size(array=w622) -> (size(s)=w621:i32)
                n237 = Greater Than 0?(x=w630) -> (x > 0?=w618:bool)
                n238 = Greater Than 0?(x=w621) -> (x > 0?=w620:bool)
                n239 = Less Than 0?(x=w634) -> (x < 0?=w594:bool)
                n240 = Strip Path(path=w604) -> (stripped path=w601:path, name=w602:string)
                n241 = Or(x=w618, y=w620) -> (x .or. y?=w619:bool)
                n242 = Not Equal?(x=w602, y="private" ("element")) -> (x != y?=w605:bool)
                n243 = Less Than 0?(x=w609) -> (x < 0?=w608:bool)
                n244 = Compound Arithmetic op=AND(w600, invert w627, w619) -> (w596:bool)
                n245 = Select(t=w604, s=w605, f=w601) -> (s? t:f=w603:path)
                n246 = Compound Arithmetic op=AND(w608, w611, w600) -> (w617:bool)
                n247 = And(x=w596, y=w594) -> (x .and. y?=w595:bool)
                n248 = case shown="True" w596 {
                  tunnel: w599 -> [w635 w638]
                  tunnel: [w635 w637] -> w597
                  tunnel: w598 -> [_ w636]
                  frame False {
                  }
                  frame True {
                    n249 = Build Array (concatenate)(w638, w636) -> (w637:path[])
                  }
                }
                n250 = case shown="True" w617 {
                  tunnel: w616 -> [w639 w642]
                  tunnel: w604 -> [_ w641]
                  tunnel: [w639 w640] -> w615
                  frame False {
                  }
                  frame True {
                    n251 = Build Array (concatenate)(w642, w641) -> (w640:path[])
                  }
                }
                n252 = case shown="True" w595 {
                  tunnel: w633 -> [w657 w660]
                  tunnel: [w657 w659] -> w632
                  tunnel: w603 -> [_ w658]
                  frame False {
                  }
                  frame True {
                    n253 = Build Array (concatenate)(w660, w658) -> (w659:path[])
                  }
                }
              }
              n254 = Bundle(cluster=w581, "Method/VI"=w583, "SubVIs/Ctls"=w584) -> (w582:T8)  [unwired: 4 in]
            }
            n255 = Bundle By Name(cluster=w575, "CreateClassVIsCalled"=w571, "dependencyClassPath"=w572, "depMethodVIs"=w569) -> (w580:T9)
          }
          frame "GetObjectAttributsDepenencies" {
            n256 = Unbundle By Name(w672) -> ("dirClass"=w663:bool, "classPath"=w661:path, "className"=w675:string)
            n257 = Concatenate Strings(w675, "ObjectAttributes.ctl" ("string")) -> (w674:string)
            n258 = case shown="True" w663 {
              tunnel: w661 -> [w677 w679]
              tunnel: [w677 w680] -> w662
              frame False {
              }
              frame True {
                n259 = Build Path(base path=w679, name or relative path="private" ("element")) -> (appended path=w680:path)
              }
            }
            n260 = Build Path(base path=w662, name or relative path=w674) -> (appended path=w667:path)
            n261 = call <resource>:"Common_GetClassAttrubutes.vi"("Path(CtrlRenumf used if Path is empty)"=w667, "error in (no error)"=w665) -> ("attributeInfo"=w664:T2[], "error out"=w666:errorcluster)  [unwired: 2 in, 14 out]
            n262 = call <resource>:"ReversedEngineering GetObjectRefsFromPanel.vi"("Path"=w667, "error in (no error)"=w666) -> ("objectRefsFound"=w669:path[], "array"=w668:bool[], "error out"=w670:errorcluster)  [unwired: 15 out]
            n263 = Bundle By Name(cluster=w672, "objectRefsInAttrib"=w669, "objectRefInAttribIsAnArray"=w668, "objectAttribInfo"=w664) -> (w673:T9)
          }
          frame "GetClassAttributsDepenencies" {
            n264 = Unbundle By Name(w693) -> ("dirClass"=w682:bool, "classPath"=w683:path, "className"=w700:string)
            n265 = Concatenate Strings(w700, "ClassAttributes.ctl" ("string")) -> (w699:string)
            n266 = case shown="True" w682 {
              tunnel: w683 -> [w701 w703]
              tunnel: [w701 w704] -> w681
              frame False {
              }
              frame True {
                n267 = Build Path(base path=w703, name or relative path="private" ("element")) -> (appended path=w704:path)
              }
            }
            n268 = Unbundle By Name(w693) -> ("objectRefsInAttrib"=w695:path[], "objectRefInAttribIsAnArray"=w690:bool[])
            n269 = Build Path(base path=w681, name or relative path=w699) -> (appended path=w687:path)
            n270 = call <resource>:"Common_GetClassAttrubutes.vi"("Path(CtrlRenumf used if Path is empty)"=w687, "error in (no error)"=w685) -> ("attributeInfo"=w684:T2[], "error out"=w686:errorcluster)  [unwired: 2 in, 14 out]
            n271 = call <resource>:"ReversedEngineering GetObjectRefsFromPanel.vi"("Path"=w687, "error in (no error)"=w686) -> ("objectRefsFound"=w692:path[], "array"=w689:bool[], "error out"=w698:errorcluster)  [unwired: 15 out]
            n272 = Build Array (concatenate)(w695, w692) -> (w696:path[])
            n273 = Build Array (concatenate)(w690, w689) -> (w691:bool[])
            n274 = Bundle By Name(cluster=w693, "objectRefsInAttrib"=w696, "objectRefInAttribIsAnArray"=w691, "classAttribInfo"=w684) -> (w694:T9)
          }
          frame "CloseRefs" {
            n275 = Unbundle By Name(w706) -> ("depClassDescRefs"=w708:refnum<vi>[])
            n276 = for {
              tunnel: w708 -> [w712] mode=indexing
              shift-right: [w710] -> w705
              shift-left: w707 -> [w711]
              n277 = call <resource>:"Common_ ViCacheMemory.vi"("ViRef"=w712, "error in (no error)"=w711) -> ("error out"=w710:errorcluster)  [unwired: 2 in, 15 out]
            }
          }
          frame "Evaluate" {
            w720 = path[] []
            # "-2 =>  2.."
            n278 = Unbundle By Name(w714) -> ("CreateClassVIsCalled"=w718:path[], "dependencyClassPath"=w722:path[], "depClassPaths"=w725:path[], "noOfObjects1"=w726:i32[], "objectAttribInfo"=w717:T2[], "classAttribInfo"=w716:T2[])
            n279 = Build Array (concatenate)(w717, w716) -> (w715:T2[])
            n280 = Unbundle By Name(w714) -> ("IsDependencyClassPathsAByValueClass"=w713:bool[])
            n281 = for {
              tunnel: w722 -> [w739] mode=indexing
              shift-right: [w756] -> w727
              shift-left: w720 -> [w757]
              shift-right: [w755] -> w728
              shift-left: w720 -> [w754]
              tunnel: w725 -> [w753]
              tunnel: w726 -> [w752]
              shift-right: [w749] -> w724
              shift-left: i32[] [] -> [w750]
              shift-right: [w746] -> w719
              shift-left: i32[] [] -> [w747]
              tunnel: w718 -> [w743]
              tunnel: w715 -> [w738]
              tunnel: w713 -> [w734]
              i -> [w733]
              # "Use minus to indicate x.."
              n282 = Search 1D Array(1D array=w753, element=w739) -> (index of element=w751:i32)  [unwired: 1 out]
              n283 = disable-structure shown="Disabled" {
                disable-tunnel: w739 -> [w758 _]
                frame Disabled {
                  n284 = call <resource>:"CommonVIs_GetClassObjectRefPath.vi"("llbClassPath"=w758) -> ()  [unwired: 17 in, 2 out]
                }
                frame Enabled {
                }
              }
              n285 = Index Array(array=w752, index=w751) -> (element=w740:i32)
              n286 = Greater Than 0?(x=w740) -> ()  [unwired: 1 out]
              n287 = Search 1D Array(1D array=w743, element=w739) -> (index of element=w742:i32)  [unwired: 1 out]
              n288 = Greater Or Equal To 0?(x=w742) -> (x >= 0?=w737:bool)
              n289 = call <resource>:"ReversedEngineering CountNoOfObjectAggregations.vi"("Path"=w739, "appended array"=w738) -> ("minAggregations"=w744:i32, "anyFound"=w748:bool, "noFoundLImit"=w745:bool)  [unwired: 1 in, 14 out]
              n290 = Index Array(array=w734, index=w733) -> (element=w732:bool)
              n291 = Or(x=w737, y=w732) -> (x .or. y?=w735:bool)
              n292 = case shown="True" w745 {
                tunnel: w744 -> [w759 w761]
                tunnel: [w759 w760] -> w736
                frame False {
                }
                frame True {
                  n293 = Negate(x=w761) -> (-x=w760:i32)
                }
              }
              n294 = And(x=w735, y=w748) -> (x .and. y?=w741:bool)
              n295 = case shown="False" w741 {
                tunnel: w757 -> [w770 w786]
                tunnel: [w770 w785] -> w756
                tunnel: w739 -> [w767 w784]
                tunnel: [w768 w783] -> w755
                tunnel: w754 -> [w769 w783]
                tunnel: w750 -> [w766 w782]
                tunnel: w736 -> [_ w781]
                tunnel: [w766 w780] -> w749
                tunnel: w748 -> [w765 _]
                tunnel: w736 -> [w764 _]
                tunnel: w747 -> [w763 w779]
                tunnel: [w762 w779] -> w746
                frame False {
                  n296 = case shown="False" w765 {
                    tunnel: w769 -> [w772 w778]
                    tunnel: [w772 w777] -> w768
                    tunnel: w767 -> [_ w776]
                    tunnel: w764 -> [_ w775]
                    tunnel: w763 -> [w771 w774]
                    tunnel: [w771 w773] -> w762
                    frame False {
                      # "Dependency"
                    }
                    frame True {
                      # "Aggregation"
                      n297 = Build Array (concatenate)(w778, w776) -> (w777:path[])
                      n298 = Build Array (concatenate)(w774, w775) -> (w773:i32[])
                    }
                  }
                }
                frame True {
                  # "Composite\nAggregation"
                  n299 = Build Array (concatenate)(w786, w784) -> (w785:path[])
                  n300 = Build Array (concatenate)(w782, w781) -> (w780:i32[])
                }
              }
            }
            n301 = Bundle By Name(cluster=w714, "compositeAggregationClassPath"=w727, "noOfCompositeObjects"=w724, "aggregationClassPath"=w728, "noOfAggObjects"=w719, "dependencyClassPath"=w722) -> (w729:T9)
          }
          frame "RemoveInheritDependency" {
            n302 = Unbundle By Name(w793) -> ("baseClasses"=w791:path[], "dependencyClassPath"=w792:path[], "compositeAggregationClassPath"=w788:path[], "aggregationClassPath"=w787:path[])
            n303 = for {
              tunnel: w792 -> [w803] mode=indexing
              tunnel: w791 -> [w806]
              shift-right: [w804] -> w789
              shift-left: path[] [] -> [w805]
              tunnel: w788 -> [w802]
              tunnel: w787 -> [w801]
              n304 = Search 1D Array(1D array=w806, element=w803) -> (index of element=w800:i32)  [unwired: 1 out]
              n305 = Search 1D Array(1D array=w802, element=w803) -> (index of element=w798:i32)  [unwired: 1 out]
              n306 = Search 1D Array(1D array=w801, element=w803) -> (index of element=w797:i32)  [unwired: 1 out]
              n307 = Compound Arithmetic op=ADD(w800, w798, w797) -> (w799:i32)
              n308 = case shown="-3" w799 {
                tunnel: w805 -> [w807 w810]
                tunnel: [w807 w809] -> w804
                tunnel: w803 -> [_ w808]
                frame Default {
                }
                frame -3 {
                  n309 = Build Array (concatenate)(w810, w808) -> (w809:path[])
                }
              }
            }
            n310 = Bundle By Name(cluster=w793, "dependencyClassPath"=w789) -> (w794:T9)
          }
          frame "CreateTypeDefs?" {
            n311 = Unbundle By Name(w812) -> ("objectAttribInfo"=w822:T2[], "classAttribInfo"=w821:T2[])
            n312 = Build Array (concatenate)(w822, w821) -> (w820:T2[])
            n313 = for {
              tunnel: w820 -> [w867] mode=indexing
              shift-right: [w868] -> w816
              shift-left: T1[] [] ("TypeDefs") -> [w864]
              n314 = Unbundle By Name(w867) -> ("type"=w866:T3, "typeName"=w853:string, "typePath"=w856:path)
              n315 = call <resource>:"Common_GetClassAttrubutes.vi"("Path(CtrlRenumf used if Path is empty)"=w856) -> ("LibraryName"=w855:string, "attributeInfo"=w862:T2[], "error out"=w861:errorcluster)  [unwired: 3 in, 13 out]
              n316 = Equal?(x=w866, y=CommonVIs_AttributeDataType."TypeDef") -> (x = y?=w860:bool)
              n317 = case shown="\"False\", Default" w855 {
                selector: w855 -> [w872 _]
                tunnel: [w869 w873] -> w854
                tunnel: w853 -> [w870 w873]
                frame "False", Default {
                  n318 = Format Into String(format string="%s : %s", w872, w870) -> (resulting string=w869:string)  [unwired: 2 in, 1 out]
                }
                frame "" {
                }
              }
              n319 = Unbundle By Name(w861) -> ("status"=w859:bool)
              n320 = Compound Arithmetic op=AND(w860, invert w859) -> (w858:bool)
              n321 = Index Array(array=w864) -> (element=w863:T1)  [unwired: 1 in]
              n322 = Bundle By Name(cluster=w863, "TypeDefName"=w854, "TypeDefPath"=w856, "TypeDefAttribInfo"=w862) -> (w857:T1)
              n323 = case shown="True" w858 {
                tunnel: w864 -> [w874 w877]
                tunnel: [w874 w876] -> w868
                tunnel: w857 -> [_ w875]
                frame False {
                }
                frame True {
                  n324 = Build Array (concatenate)(w877, w875) -> (w876:T1[])
                }
              }
            }
            n325 = for {
              tunnel: w816 -> [w827] mode=indexing
              shift-right: [w824] -> w814
              shift-left: T1[] [] ("TypeDefs") -> [w825]
              n326 = Unbundle By Name(w827) -> ("TypeDefAttribInfo"=w826:T2[])
              n327 = for {
                tunnel: w826 -> [w842] mode=indexing
                shift-right: [w843] -> w824
                shift-left: w825 -> [w839]
                n328 = Unbundle By Name(w842) -> ("type"=w841:T3, "typeName"=w829:string, "typePath"=w831:path)
                n329 = Equal?(x=w841, y=CommonVIs_AttributeDataType."TypeDef") -> (x = y?=w835:bool)
                n330 = call <resource>:"Common_GetClassAttrubutes.vi"("Path(CtrlRenumf used if Path is empty)"=w831) -> ("LibraryName"=w830:string, "attributeInfo"=w837:T2[], "error out"=w836:errorcluster)  [unwired: 3 in, 13 out]
                n331 = case shown="\"False\", Default" w830 {
                  selector: w830 -> [w847 _]
                  tunnel: [w844 w848] -> w828
                  tunnel: w829 -> [w845 w848]
                  frame "False", Default {
                    n332 = Format Into String(format string="%s : %s", w847, w845) -> (resulting string=w844:string)  [unwired: 2 in, 1 out]
                  }
                  frame "" {
                  }
                }
                n333 = Unbundle By Name(w836) -> ("status"=w834:bool)
                n334 = Compound Arithmetic op=AND(w835, invert w834) -> (w833:bool)
                n335 = Index Array(array=w839) -> (element=w838:T1)  [unwired: 1 in]
                n336 = Bundle By Name(cluster=w838, "TypeDefName"=w828, "TypeDefPath"=w831, "TypeDefAttribInfo"=w837) -> (w832:T1)
                n337 = case shown="True" w833 {
                  tunnel: w839 -> [w849 w852]
                  tunnel: [w849 w851] -> w843
                  tunnel: w832 -> [_ w850]
                  frame False {
                  }
                  frame True {
                    n338 = Build Array (concatenate)(w852, w850) -> (w851:T1[])
                  }
                }
              }
            }
            n339 = Unbundle By Name(w812) -> ("TypeDefs"=w811:T1[])
            n340 = Build Array (concatenate)(w811, w816, w814) -> (w813:T1[])
            n341 = Bundle By Name(cluster=w812, "TypeDefs"=w813) -> (w819:T9)
          }
          frame "AddReferencedTypeDefs" {
            n342 = Unbundle By Name(w885) -> ("TypeDefs"=w878:T1[], "depMethodVIs"=w880:T8[])
            n343 = for {
              tunnel: w878 -> [w887] mode=indexing
              tunnel: [w886] -> w879 mode=indexing
              n344 = Unbundle By Name(w887) -> ("TypeDefPath"=w886:path)
            }
            n345 = for {
              shift-right: [w889] -> w882
              shift-left: w878 -> [w888]
              tunnel: w880 -> [w895] mode=indexing
              shift-right: [w892] -> _
              shift-left: w879 -> [w893]
              n346 = Unbundle By Name(w895) -> ("SubVIs/Ctls"=w894:path[], "SubVIClassOwner"=w891:string[], "ClassMethodName"=w890:string[])
              n347 = for {
                tunnel: w894 -> [w898] mode=indexing
                shift-right: [w903] -> w889
                shift-left: w888 -> [w904]
                shift-right: [w902] -> w892
                shift-left: w893 -> [w905]
                tunnel: w891 -> [w901] mode=indexing
                tunnel: w890 -> [w900] mode=indexing
                n348 = Strip Path(path=w898) -> (stripped path=w897:path)  [unwired: 1 out]
                n349 = call <vilib>:"Get File Extension.vi"("file"=w897) -> ("lowercase file extension"=w896:string)  [unwired: 1 in, 9 out]
                n350 = call <vilib>:"Get File Extension.vi"("file"=w898) -> ("filename without extension"=w899:string, "lowercase file extension"=w907:string, "dup file"=w906:path)  [unwired: 1 in, 7 out]
                n351 = case shown="\"ctl\", \"ctt\"" w907 {
                  tunnel: w906 -> [_ w912]
                  tunnel: w905 -> [w908 w915]
                  tunnel: w904 -> [w909 w916]
                  tunnel: [w909 w914] -> w903
                  tunnel: [w908 w913] -> w902
                  tunnel: w901 -> [_ _]
                  tunnel: w900 -> [_ _]
                  tunnel: w899 -> [_ w911]
                  tunnel: w896 -> [_ w910]
                  frame "False", Default {
                  }
                  frame "ctl", "ctt" {
                    n352 = case shown="\"lvclass\"" w910 {
                      tunnel: w916 -> [w918 w924]
                      tunnel: w915 -> [w917 w923]
                      tunnel: [w918 w922] -> w914
                      tunnel: [w917 w921] -> w913
                      tunnel: w912 -> [_ w920]
                      tunnel: w911 -> [_ w919]
                      frame "lvclass" {
                      }
                      frame Default {
                        n353 = Search 1D Array(1D array=w923, element=w920) -> (index of element=w925:i32)  [unwired: 1 out]
                        n354 = case shown="-1" w925 {
                          tunnel: w924 -> [w927 w942]
                          tunnel: w923 -> [w926 w940]
                          tunnel: [w927 w941] -> w922
                          tunnel: [w926 w939] -> w921
                          tunnel: w920 -> [_ w934]
                          tunnel: w919 -> [_ w936]
                          frame 0, Default {
                          }
                          frame -1 {
                            n355 = call <resource>:"Common_GetClassAttrubutes.vi"("Path(CtrlRenumf used if Path is empty)"=w934) -> ("LibraryName"=w933:string, "attributeInfo"=w932:T2[], "error out"=w931:errorcluster)  [unwired: 3 in, 13 out]
                            n356 = case shown="\"False\", Default" w933 {
                              selector: w933 -> [w954 _]
                              tunnel: [w951 w955] -> w935
                              tunnel: w936 -> [w952 w955]
                              frame "False", Default {
                                n357 = Format Into String(format string="%s : %s", w954, w952) -> (resulting string=w951:string)  [unwired: 2 in, 1 out]
                              }
                              frame "" {
                              }
                            }
                            n358 = Unbundle(w931) -> ("status"=w929:bool)  [unwired: 2 out]
                            n359 = Empty Array?(array=w932) -> (empty?=w930:bool)
                            n360 = Or(x=w930, y=w929) -> (x .or. y?=w928:bool)
                            n361 = Bundle(cluster=T1 {"TypeDefName"="", "TypeDefPath"=path "", "TypeDefAttribInfo"=[]} ("TypeDef"), "TypeDefName"=w935, "TypeDefPath"=w934, "TypeDefAttribInfo"=w932) -> (w937:T1)
                            n362 = case shown="False" w928 {
                              tunnel: w942 -> [w948 w950]
                              tunnel: [w947 w950] -> w941
                              tunnel: w940 -> [w946 w949]
                              tunnel: [w945 w949] -> w939
                              tunnel: w937 -> [w944 _]
                              tunnel: w934 -> [w943 _]
                              frame False {
                                n363 = Build Array (concatenate)(w948, w944) -> (w947:T1[])
                                n364 = Build Array (concatenate)(w946, w943) -> (w945:path[])
                              }
                              frame True {
                              }
                            }
                          }
                        }
                      }
                    }
                  }
                }
              }
            }
            n365 = Bundle By Name(cluster=w885, "TypeDefs"=w882) -> (w884:T9)
          }
          frame "UpdateTypeDefsAttribName?" {
            n366 = Unbundle By Name(w965) -> ("objectAttribInfo"=w962:T2[], "classAttribInfo"=w960:T2[], "TypeDefs"=w957:T1[])
            n367 = for {
              tunnel: w957 -> [w968] mode=indexing
              tunnel: [w966] -> w956 mode=indexing
              n368 = Unbundle By Name(w968) -> ("TypeDefAttribInfo"=w969:T2[])
              n369 = for {
                tunnel: w969 -> [w972] mode=indexing
                tunnel: [w971] -> w967 mode=indexing
                n370 = Unbundle By Name(w972) -> ("type"=w979:T3, "typeName"=w976:string)
                n371 = Equal?(x=w979, y=CommonVIs_AttributeDataType."TypeDef") -> (x = y?=w973:bool)
                n372 = String To Path(string=w976) -> (path=w974:path)
                n373 = Strip Path(path=w974) -> (name=w977:string)  [unwired: 1 out]
                n374 = Match Pattern(string=w977, regular expression="[.][cC][tT][lL]$") -> (before substring=w970:string)  [unwired: 4 out]
                n375 = case shown="True" w973 {
                  tunnel: w972 -> [w980 w983]
                  tunnel: [w980 w982] -> w971
                  tunnel: w970 -> [_ w981]
                  frame False {
                  }
                  frame True {
                    n376 = Bundle By Name(cluster=w983, "typeName"=w981) -> (w982:T2)
                  }
                }
              }
              n377 = Bundle By Name(cluster=w968, "TypeDefAttribInfo"=w967) -> (w966:T1)
            }
            n378 = for {
              tunnel: w962 -> [w1000] mode=indexing
              tunnel: [w999] -> w961 mode=indexing
              n379 = Unbundle By Name(w1000) -> ("type"=w1007:T3, "typeName"=w1004:string)
              n380 = Equal?(x=w1007, y=CommonVIs_AttributeDataType."TypeDef") -> (x = y?=w1001:bool)
              n381 = String To Path(string=w1004) -> (path=w1002:path)
              n382 = Strip Path(path=w1002) -> (name=w1005:string)  [unwired: 1 out]
              n383 = Match Pattern(string=w1005, regular expression="[.][cC][tT][lL]$") -> (before substring=w998:string)  [unwired: 4 out]
              n384 = case shown="True" w1001 {
                tunnel: w1000 -> [w1008 w1011]
                tunnel: [w1008 w1010] -> w999
                tunnel: w998 -> [_ w1009]
                frame False {
                }
                frame True {
                  n385 = Bundle By Name(cluster=w1011, "typeName"=w1009) -> (w1010:T2)
                }
              }
            }
            n386 = for {
              tunnel: w960 -> [w986] mode=indexing
              tunnel: [w985] -> w959 mode=indexing
              n387 = Unbundle By Name(w986) -> ("type"=w993:T3, "typeName"=w990:string)
              n388 = Equal?(x=w993, y=CommonVIs_AttributeDataType."TypeDef") -> (x = y?=w987:bool)
              n389 = String To Path(string=w990) -> (path=w988:path)
              n390 = Strip Path(path=w988) -> (name=w991:string)  [unwired: 1 out]
              n391 = Match Pattern(string=w991, regular expression="[.][cC][tT][lL]$") -> (before substring=w984:string)  [unwired: 4 out]
              n392 = case shown="True" w987 {
                tunnel: w986 -> [w994 w997]
                tunnel: [w994 w996] -> w985
                tunnel: w984 -> [_ w995]
                frame False {
                }
                frame True {
                  n393 = Bundle By Name(cluster=w997, "typeName"=w995) -> (w996:T2)
                }
              }
            }
            n394 = Bundle By Name(cluster=w965, "objectAttribInfo"=w961, "classAttribInfo"=w959, "TypeDefs"=w956) -> (w964:T9)
          }
          frame "SortMethodToClassDependencies" {
            w1014 = cluster{path[]}[] []
            n395 = Unbundle By Name(w1021) -> ("depMethodVIs"=w1018:T8[])
            n396 = for {
              shift-right: [w1043] -> w1020
              shift-left: path[] [] -> [w1045]
              shift-right: [w1042] -> w1016
              shift-left: w1014 -> [w1039]
              tunnel: w1018 -> [w1046] mode=indexing
              shift-right: [w1040] -> w1015
              shift-left: w1014 -> [w1038]
              shift-right: [w1036] -> w1012
              shift-left: cluster{T7[]}[] [] -> [w1034]
              n397 = Unbundle(w1046) -> ("Method/VI"=w1041:path, "SubVIs/Ctls"=w1044:path[], "SubVIClassOwnerPath"=w1037:path[], "DepType"=w1035:T7[])  [unwired: 2 out]
              n398 = for {
                shift-right: [w1059] -> w1043
                shift-left: w1045 -> [w1058]
                tunnel: w1044 -> [w1051] mode=indexing
                shift-right: [w1055] -> w1042
                shift-left: w1039 -> [w1056]
                tunnel: w1041 -> [w1054]
                shift-right: [w1053] -> w1040
                shift-left: w1038 -> [w1052]
                tunnel: w1037 -> [w1050] mode=indexing
                shift-right: [w1048] -> w1036
                shift-left: w1034 -> [w1049]
                tunnel: w1035 -> [w1047] mode=indexing
                # "ConvertTo\nClassPath"
                n399 = Search 1D Array(1D array=w1058, element=w1050) -> (index of element=w1057:i32)  [unwired: 1 out]
                n400 = case shown="Default" w1057 {
                  selector: w1057 -> [w1060 _]
                  tunnel: [w1082 w1098] -> w1059
                  tunnel: w1050 -> [_ w1100]
                  tunnel: w1058 -> [w1082 w1099]
                  tunnel: w1056 -> [w1077 w1095]
                  tunnel: [w1076 w1094] -> w1055
                  tunnel: w1054 -> [w1079 w1093]
                  tunnel: w1052 -> [w1069 w1090]
                  tunnel: [w1070 w1091] -> w1053
                  tunnel: w1051 -> [w1068 w1092]
                  tunnel: w1049 -> [w1066 w1085]
                  tunnel: [w1065 w1084] -> w1048
                  tunnel: w1047 -> [w1067 w1083]
                  frame Default {
                    n401 = Index Array(array=w1077, index=w1060) -> (element=w1081:cluster{path[]})
                    n402 = Index Array(array=w1069, index=w1060) -> (element=w1071:cluster{path[]})
                    n403 = Index Array(array=w1066, index=w1060) -> (element=w1064:cluster{T7[]})
                    n404 = Unbundle(w1081) -> (w1080:path[])
                    n405 = Unbundle(w1071) -> (w1072:path[])
                    n406 = Unbundle(w1064) -> (w1063:T7[])
                    n407 = Build Array (concatenate)(w1080, w1079) -> (w1078:path[])
                    n408 = Build Array (concatenate)(w1072, w1068) -> (w1073:path[])
                    n409 = Build Array (concatenate)(w1063, w1067) -> (w1062:T7[])
                    n410 = Bundle(w1078) -> (w1075:cluster{path[]})  [unwired: 1 in]
                    n411 = Bundle(w1073) -> (w1074:cluster{path[]})  [unwired: 1 in]
                    n412 = Bundle(w1062) -> (w1061:cluster{T7[]})  [unwired: 1 in]
                    n413 = Replace Array Subset(array=w1077, new element=w1075, index=w1060) -> (w1076:cluster{path[]}[])
                    n414 = Replace Array Subset(array=w1069, new element=w1074, index=w1060) -> (w1070:cluster{path[]}[])
                    n415 = Replace Array Subset(array=w1066, new element=w1061, index=w1060) -> (w1065:cluster{T7[]}[])
                  }
                  frame -1 {
                    n416 = Build Array(w1093) -> (w1096:path[])
                    n417 = Build Array(w1092) -> (w1089:path[])
                    n418 = Bundle(w1096) -> (w1097:cluster{path[]})  [unwired: 1 in]
                    n419 = Bundle(w1089) -> (w1088:cluster{path[]})  [unwired: 1 in]
                    n420 = Build Array(w1083) -> (w1086:T7[])
                    n421 = Build Array (concatenate)(w1099, w1100) -> (w1098:path[])
                    n422 = Build Array (concatenate)(w1095, w1097) -> (w1094:cluster{path[]}[])
                    n423 = Build Array (concatenate)(w1090, w1088) -> (w1091:cluster{path[]}[])
                    n424 = Bundle(w1086) -> (w1087:cluster{T7[]})  [unwired: 1 in]
                    n425 = Build Array (concatenate)(w1085, w1087) -> (w1084:cluster{T7[]}[])
                  }
                }
              }
            }
            n426 = for {
              tunnel: w1020 -> [w1032] mode=indexing
              tunnel: [w1030] -> w1019 mode=indexing
              tunnel: w1016 -> [w1029] mode=indexing
              tunnel: w1015 -> [w1028] mode=indexing
              tunnel: w1012 -> [w1026] mode=indexing
              n427 = Unbundle(w1029) -> (w1031:path[])
              n428 = Unbundle(w1028) -> (w1027:path[])
              n429 = Unbundle(w1026) -> (w1025:T7[])
              n430 = Bundle(cluster=T6 {"DepClassPath"=path "", "ThisVIs/Ctls"=[], "Dependent_VIs/Ctls"=[], "ViDependecyType"=[]} ("DepClass"), "DepClassPath"=w1032, "ThisVIs/Ctls"=w1031, "Dependent_VIs/Ctls"=w1027, "ViDependecyType"=w1025) -> (w1030:T6)
            }
            n431 = Bundle By Name(cluster=w1021, "DependencyDetails"=w1019) -> (w1023:T9)
          }
          frame "Error", Default {
          }
        }
        n432 = call <resource>:"UMLEditor ControlBusyDialog.vi"("error in (no error)"=w52, "Action(SendStatusMessage)"=w51) -> ("error out"=w48:errorcluster)  [unwired: 2 in, 15 out]
        n433 = Equal?(x=w61, y="Exit") -> (x = y?=w59:bool)
        n434 = Or(x=w59, y=w48) -> (x .or. y?=w58:bool)
      }
    }
    frame Error {
    }
  }
  n435 = Unbundle By Name(w30) -> ("TypeDefs"=→"TypeDefs":T1[], "inherits"=w27:bool, "baseClasses"=w26:path[], "compositeAggregationClassPath"=w25:path[], "noOfCompositeObjects"=w24:i32[], "aggregationClassPath"=w23:path[], "noOfAggObjects"=w22:i32[], "dependencyClassPath"=w21:path[], "methodNames"=w20:string[], "methodPuplic"=w19:T4[], "objectAttribInfo"=w18:T2[], "classAttribInfo"=w17:T2[], "ClassDesc"=w10:string, "DependencyDetails"=w7:T6[], "Interface"=w3:bool, "ParentInterfaces"=w2:path[], "createRef"=w9:refnum<vi>, "errMsg"=w13:string)
  n436 = case shown="Error" w16 {
    selector: w16 -> [w1105 w1113]
    tunnel: [w1105 w1112] -> w15
    tunnel: w14 -> [_ w1109]
    tunnel: w13 -> [_ w1107]
    frame No Error {
    }
    frame Error {
      n437 = Unbundle By Name(w1113) -> ("code"=w1106:i32, "source"=w1108:string)
      n438 = Format Into String(format string="<ERR>\nCase:%s\nError:[%d]%s\nSource:%s", w1109, w1106, w1107, w1108) -> (resulting string=w1110:string)  [unwired: 2 in, 1 out]
      n439 = Bundle By Name(cluster=w1113, "source"=w1110) -> (w1112:errorcluster)
    }
  }
  "error out" <- w15
  n440 = call <resource>:"Common_ ViCacheMemory.vi"("ViRef"=w9) -> ()  [unwired: 3 in, 16 out]
  n441 = local read "classInfo"() -> (w29:T5)
  n442 = Bundle By Name(cluster=w29, "classPath"="Class/Create Path", "inherits"=w27, "baseClasses"=w26, "compAggClasses"=w25, "noOfCompObj"=w24, "aggClasses"=w23, "noOfAgg"=w22, "depClasses"=w21, "methods"=w20, "methodPuplic"=w19, "objectAttrib"=w18, "classAttrib"=w17, "ClassDesc"=w10, "DependencyDetails"=w7, "Interface"=w3, "ParentInterfaces"=w2) -> (→"classInfo":T5)
